vi "20180801 2nd Step Analysis.vi"(8 "error in":errorcluster caption="エラー入力（エラーなし）", 9 "Numeric":i32=5, 10 "S New Info and MiN":T28={"Sample Sequence"="GATGATGATGATGATGAT", "Right Read MIN"=6, "Filter P"=0, "STD Type"=enum."Region", "Base Table"=[], "Selection"=enum."10kHz", "noise MAX"=3, "Sample name"="(GAT)x6"} {"Base Table"."Value 3" format="%.2g"}, 11 "Filename":path) -> (0 "error out":errorcluster caption="エラー出力", 2 "Raw data Graph":dbl[](graph), 3 "Total NGraph_MS":dbl[][](graph))   [LabVIEW 2018]
uses:
  VI/control1.ctl
  <vilib>/Analysis/NI_AALBase.lvlib
panel:
  out "error out 3":errorcluster
  out "FN#":string
  out "Array":string[](array[string])
  out "error out 2":errorcluster caption="エラー出力"
  in  "target path (use dialog)":path
  out "B_TDMS_Path_Temp":path
  out "MS_Total Con and T":cluster{dbl[], dbl[], dbl[], dbl[], i32[]}
  out "Plot Graph":dbl[][](graph)
  out "Base_Tag_Array":string[](array[string])
  out "Base_Com_Array":i32[](array[numeric])
  out "Total C Plot_MS":dbl[][](array[numeric])
  out "R Con H_MS":dbl[][](array[numeric])
  out "LCPZ":T1
  out "LCPX_CZ":T1
  out "LCPX_C2":T2
  out "LAP Table":string[][](table) caption="LCP Table"
  out "Table cluster_B":T3
  out "LSP_C2":T4
  out "LSPX_C1":T5
  out "LCPX_C1":T6
  out "Assigned#_CL":T4
  out "AR BN#":i32[](array[numeric])
  out "Long Signal#":i32
  out "AR T#":i32
  in  "B_END [s]":dbl format="%#_13g"
  in  "B_Start [s]":dbl format="%#_13g"
  in  "Tag cluster_B":T7
  out "LTP Table":string[][](table) caption="LS Table"
  out "LTP Table Tag":string[](array[string])
  out "LTP Table Pass":path
  out "MxRight_Array":string[](array[string])
  out "Assigned_Array":string[](array[string])
  out "LSP_C2":T8
  out "LSP_C1":T9
  in  "LCP_C1":T10
  out "LCP Table CSV refnum":refnum<file>
  out "LSP Table CSV refnum":refnum<file>
  out "LSP Table":string[][](table) caption="LS Table"
  out "LCP Table":string[][](table) caption="CP Table"
  out "LCP Table Tag":string[](array[string])
  out "LSP Table Tag":string[](array[string])
  out "LCP Table Pass":path
  out "LSP Table Pass":path
  out "after":string
  out "BNAL TD":T11
  out "BNAL Program Date":string
  out "B prep":T12
  out "BNAL Program":string
  out "TDMS Tpath":refnum<k34>
  out "AR Table":string[][](array[string])
  out "AR Table Tag":string[](array[string])
  out "S Table Tag":string[](array[string])
  out "B_TDMS_Path":path
  out "B_TDMS Path":string
  out "BR time [s]":dbl
  out "assembly C":T13 {"Assembly Ratio" format="%#.2g"}
  out "GAF":T14
  in  "noise MAX":i32=3
  out "AR#":i32[](array[numeric])
  out "RR#":i32[](array[numeric])
  out "Anal Time":string
  out "1s datapoint":i32
  in  "Selection":enum16{"10kHz", "100kHz"}(ring)
  out "BR all info":T15
  out "B info":string[](array[string])
  out "AC Table Tag":string[](array[string])
  out "R Table Tag":string[](array[string])
  out "R Con H":dbl[][](array[numeric])
  out "BC1":cluster{"B region#":i32, "Date":string}
  out "BNAL Path":T16
  out "LS Path":T17
  out "Total C Plot":dbl[][](graph)
  out "Folder Path":string
  out "Date":string
  out "Base R Level":dbl[](array[numeric])
  out "Base A Level":dbl[](array[numeric])
  out "Base Color":u32[](array[numeric])
  out "Level Composition":string[](array[string])
  out "Base Ex Info":T18
  out "Total Con and T":T19
  out "CP A Tag AZ":string[](array[string])
  out "Time A Table AZ":string[](array[string])
  out "BS Table Tag":string[](array[string])
  out "BS Table":string[][](table) caption="S Table"
  out "GR data":T20
  out "Selected Raw D":T21
  in  "Control_2":T22(tab)
  out "Time Graph":cluster{"time":dbl[], "current":dbl[]}[](graph)
  out "Time Graph Profile":cluster{"time":dbl[], dbl[]}[](graph)
  out "Label":T23
  out "CP Graph":cluster{i32[], dbl[]}[](graph)
  out "CP Graph Profile":cluster{i32[], dbl[]}[](graph)
  out "Label 2":T23
  out "Signal# Histogram":cluster{"配列 2":i32[], "配列 5":dbl[]}[](graph)
  out "Long Assembly":bool[][](array[boolean])
  out "Total assembly C":T24 {"Assembly Ratio 2" format="%#_3g"; "Assembly Ratio" format="%#_3g"}
  out "Total BC":bool[](array[boolean])
  out "RR#":i32
  out "S#":i32
  out "Av R_Read N":dbl format="%#_4g"
  out "Av N_Read N":dbl format="%#_4g"
  out "Covered?":bool
  out "MAX RR#":i32
  out "coverage [%]":dbl format="%#.2g"
  out "5’→3'":dbl format="%#.3g"
  out "Total Base CP":i32
  out "RR MIN Over S#":i32
  out "SB_ANA":T25
  out "Av n#bp":i32
  out "Av RR n#bp":i32
  out "Av RRn# kbp/day":dbl format="%#_3f"
  out "Av n# kbp/day":dbl format="%#_3f"
  out "Total AGraph":dbl[][](graph)
  out "Q_Histogram":T26(graph)
  out "Time Histogram":T26(graph)
  out "I Histogram":T26(graph) caption="I_Histogram"
  out "Total NGraph":dbl[][](graph)
  out "Count Graph":cluster{i32[], i32[]}(graph) caption="ヒストグラムグラフ"
  out "Cutted Sample Sequence":string
  out "MS_Count Graph":cluster{i32[], i32[]}(graph) caption="ヒストグラムグラフ"
  out "Sample Sequence":string
  out "All Radar_X":picture
  out "All Radar Plot_XX":picture
  out "Mono Table":string[][](table)
  out "Di Table":string[][](table)
  out "Tri Table":string[][](table)
  out "Base Species (n)":i32
  out "Right Read MIN":i32
  out "Base (n)":i32
  in  "Control_1":T27(tab)
  in  "Locked":bool=TRUE
  out "before":string
  out "B Table":string[][](table)
  out "R Table":string[][](table)
  out "Data Histogram":T26(graph) caption="ヒストグラムグラフ"
  out "Label 3":T23
  out "AC Table":T29
  out "Progress":dbl(slide) scale=0.0..100.0
  out "B_Region#":i32
  out "Total B Region#":i32
  out "Channel Tag":string[](array[string])
  out "Table Tag":string[][](array[string])
  out "B End [s]":dbl[](array[numeric])
  out "B Start [s]":dbl[](array[numeric])
  out "B Table Tag":string[](array[string])
  out "Raw data":dbl[](array[numeric])
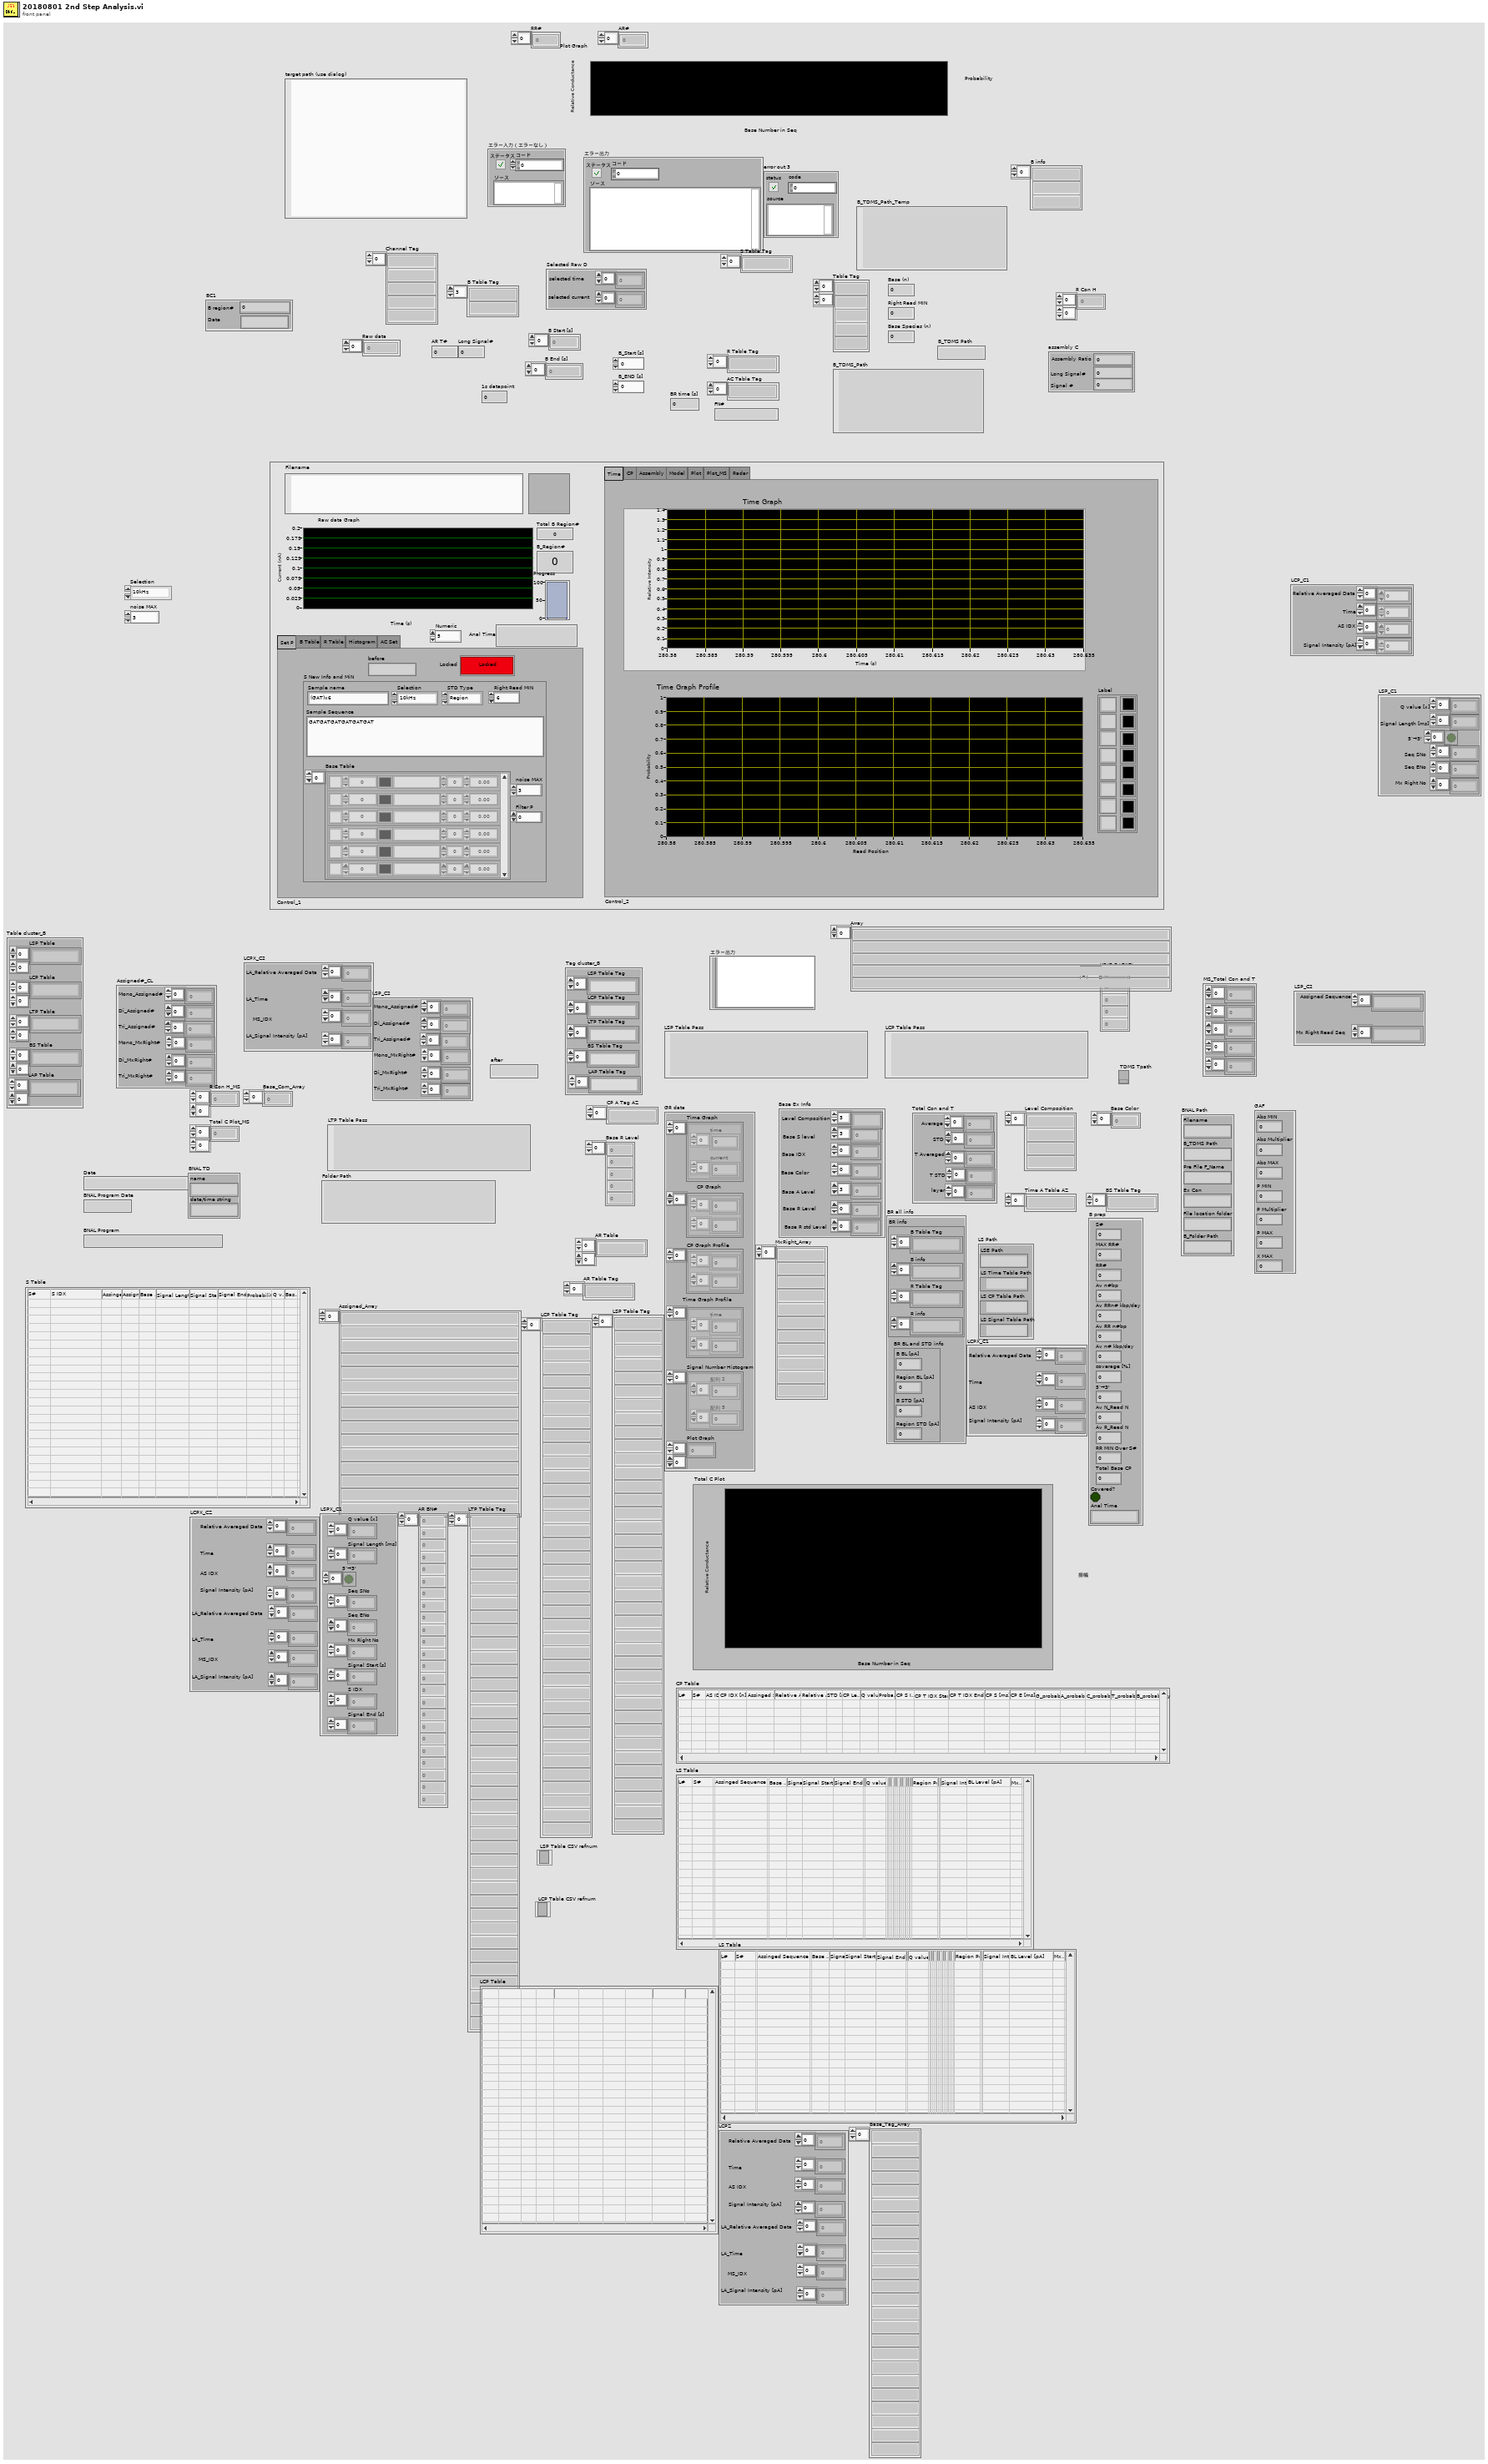
[diagram p1: front panel]
types:
  T1 = cluster{"Relative Averaged Data":dbl[], "Time":dbl[], "AS IDX":i32[], "Signal Intensity [pA]":dbl[], "LA_Relative Averaged Data":dbl[], "LA_Time":dbl[], "MS_IDX":i32[], "LA_Signal Intensity [pA]":dbl[]}
  T2 = cluster{"LA_Relative Averaged Data":dbl[], "LA_Time":dbl[], "MS_IDX":i32[], "LA_Signal Intensity [pA]":dbl[]}
  T3 = cluster{"LSP Table":string[][], "LCP Table":string[][], "LTP Table":string[][], "BS Table":string[][], "LAP Table":string[][]}
  T4 = cluster{"Mono_Assigned#":i32[], "Di_Assigned#":i32[], "Tri_Assigned#":i32[], "Tri_MxRight#":i32[], "Di_MxRight#":i32[], "Mono_MxRight#":i32[]}
  T5 = cluster{"Q value [x]":dbl[], "Signal Length [ms]":dbl[], "5’→3'":bool[], "Seq SNo":i32[], "Seq ENo":i32[], "Mx Right No":i32[], "Signal Start [s]":dbl[], "S IDX":i32[], "Signal End [s]":dbl[]}
  T6 = cluster{"Relative Averaged Data":dbl[], "Time":dbl[], "AS IDX":i32[], "Signal Intensity [pA]":dbl[]}
  T7 = cluster{"LSP Table Tag":string[], "LCP Table Tag":string[], "LTP Table Tag":string[], "BS Table Tag":string[], "LAP Table Tag":string[]}
  T8 = cluster{"Assigned Sequence":string[], "Mx Right Read Seq":string[]}
  T9 = cluster{"Q value [x]":dbl[], "Signal Length [ms]":dbl[], "5’→3'":bool[], "Seq SNo":i32[], "Seq ENo":i32[], "Mx Right No":i32[]}
  T10 = cluster{"Relative Averaged Data":dbl[], "Time":dbl[], i32[], "Signal Intensity [pA]":dbl[]}
  T11 = cluster{"name":string, "date/time string":string}
  T12 = cluster{"S#":i32, "MAX RR#":i32, "RR#":i32, "Av n#bp":i32, "Av RRn# kbp/day":dbl, "Av RR n#bp":i32, "Av n# kbp/day":dbl, "coverage [%]":dbl, "5’→3'":dbl, "Av N_Read N":dbl, "Av R_Read N":dbl, "RR MIN Over S#":i32, "Total Base CP":i32, "Covered?":bool, "Anal Time":string}
  T13 = cluster{"Assembly Ratio":dbl, "Long Signal#":i32, "Signal #":i32}
  T14 = cluster{"Abs MIN":dbl, "Abs Multiplier":dbl, "Abs MAX":dbl, "P MIN":dbl, "P Multiplier":dbl, "P MAX":dbl, "X MAX":dbl}
  T15 = cluster{"BR info":cluster{"B Table Tag":string[], "B info":string[], "R Table Tag":string[], "R info":string[]}, "BR BL and STD info":cluster{"B BL [pA]":dbl, "Region BL [pA]":dbl, "B STD [pA]":dbl, "Region STD [pA]":dbl}}
  T16 = cluster{"Filename":string, "B_TDMS Path":string, "Pre File F_Name":string, "Ex Con":string, "File location folder":string, "B_Folder Path":string}
  T17 = cluster{"LSE Path":string, "LS Time Table Path":path, "LS CP Table Path":path, "LS Signal Table Path":path}
  T18 = cluster{"Level Composition":string[], "Base S level":dbl[], "Base IDX":i32[], "Base Color":u32[], "Base A Level":dbl[], "Base R Level":dbl[], "Base R std Level":dbl[]}
  T19 = cluster{"Average":dbl[], "STD":dbl[], "T Averaged":dbl[], "T STD":dbl[], "layer":i32[]}
  T20 = cluster{"Time Graph":cluster{"time":dbl[], "current":dbl[]}[], "CP Graph ":cluster{i32[], dbl[]}[], "CP Graph Profile":cluster{i32[], dbl[]}[], "Time Graph Profile":cluster{"time":dbl[], dbl[]}[], "Signal Number Histogram":cluster{"配列 2":i32[], "配列 5":dbl[]}[], "Plot Graph":dbl[][]}
  T21 = cluster{"selected time":dbl[], "selected current":dbl[]}
  T22 = enum32{"Time", "CP", "Assembly", "Model", "Plot", "Plot_MS", "Radar"}
  T23 = cluster{"カラーボックス":u32, "カラーボックス 4":u32, "カラーボックス 2":u32, "カラーボックス 5":u32, "カラーボックス 3":u32, "カラーボックス 6":u32, "カラーボックス 7":u32, "カラーボックス 8":u32, "B0":string, "B1":string, "B2":string, "B3":string, "B4":string, "B5":string, "B6":string, "B7":string}
  T24 = cluster{"Assembly Ratio":dbl, "Long Signal#":i32, "Signal #":i32, "Assembly Ratio 2":dbl}
  T25 = cluster{"RR Ratio (%)":dbl, "Base Species#":i32, "RR option#":i32, "all option#":i32, "RRS#":i32, "Base Cutted Q#":i32}
  T26 = cluster{"X Values":dbl[], "Histogram: h(x)":i32[]}
  T27 = enum32{"Set P", "B Table", "R Table", "Histogram", "AC Set"}
  T28 = cluster{"Sample Sequence":string, "Right Read MIN":i32, "Filter P":i32, "STD Type":enum16{"Region", "Each", "Fixed"}, "Base Table":cluster{"Name":string, "Value":dbl, "Color":u32, "Name 2":string, "Value 2":dbl, "Value 3":dbl}[], "Selection":enum16{"10kHz", "100kHz"}, "noise MAX":i32, "Sample name":string}
  T29 = typedef "control1.ctl" = string[][]
  T30 = cluster{"Relative Averaged Data":dbl[], "Time":dbl[], "AS IDX":i32[], "Abs Average":dbl[]}
  T31 = enum16{"open", "open or create", "create or replace", "create", "open (read-only)"}
  T32 = cluster{"Name":string, "Value":dbl, "Color":u32, "Name 2":string, "Value 2":dbl, "Value 3":dbl}[]
  T33 = cluster{"Base Composition":string[], "Base S Level":dbl[], "Color IDX":u32[], "Base ex Composition":string[], "Base IDX":i32[], "STD S Level [pA]":dbl[]}
  T34 = cluster{"Assembly Ratio":dbl, "Assembly Ratio":i32, "Assembly Ratio":i32, "Assembly Ratio":dbl}
  T35 = cluster{"LSP Table Pass":path, "LCP Table Pass":path, "LTP Table Pass":path}
  T36 = cluster{"Data Estimated Info":cluster{"Mx level":dbl, "Mx Level Intensity":dbl, "BL Level":dbl, "MAX":dbl, "Min":dbl, "Histogram bin":dbl, "Region Cut":dbl, "Data Point":i32, "Filename":string, "G level intensity":dbl}, "Base Ex Info":cluster{"Level Composition":string[], "Base S level":dbl[], "Base IDX":i32[], "Base Color":u32[], "Base A Level":dbl[], "Base R Level":dbl[], "Base R std Level":dbl[]}}
  T37 = cluster{"Assigned Sequence":string[], "L#":i32[], "Mx Right Read Seq":string[], "Base Number":i32[], "Signal Intensity [pA]":dbl[]}
  T38 = cluster{"Count Graph":cluster{i32[], i32[]}, "Total Con and T":cluster{dbl[], dbl[], dbl[], dbl[], i32[]}, "GAT":cluster{"Value":cluster{"Abs MIN":dbl, "Abs Multiplier":dbl, "Abs MAX":dbl, "P MIN":dbl, "P Multiplier":dbl, "P MAX":dbl, "X MAX":dbl}, "Axis":dbl[], "Axis":dbl[]}}
  T39 = cluster{"Plot Graph":dbl[][], "N_Grpah":dbl[][], "Abs_Graph":dbl[][]}
  T40 = cluster{"Value":cluster{"Abs MIN":dbl, "Abs Multiplier":dbl, "Abs MAX":dbl, "P MIN":dbl, "P Multiplier":dbl, "P MAX":dbl, "X MAX":dbl}, "Axis":dbl[], "Axis":dbl[]}
  T41 = cluster{"Mono Table":string[][], "Mono Table":string[][], "Mono Table":string[][]}
  T42 = cluster{"Radar Plot":picture, "Radar Plot":picture, "Radar Plot":picture}
  T43 = cluster{"Value":i32, "Value":i32, "Value":i32, "Value":i32, "Value":dbl, "Value":i32, "Value":dbl, "Value":dbl, "Value":dbl, "Value":dbl, "Value":dbl, "Value":i32, "Value":i32, "Value":bool, "Value":string}
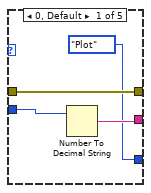
[diagram p3: hidden frame]
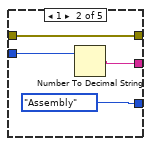
[diagram p4: hidden frame]
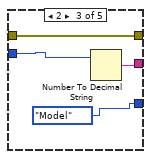
[diagram p5: hidden frame]
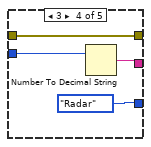
[diagram p6: hidden frame]
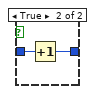
[diagram p7: hidden frame]
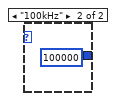
[diagram p9: hidden frame]
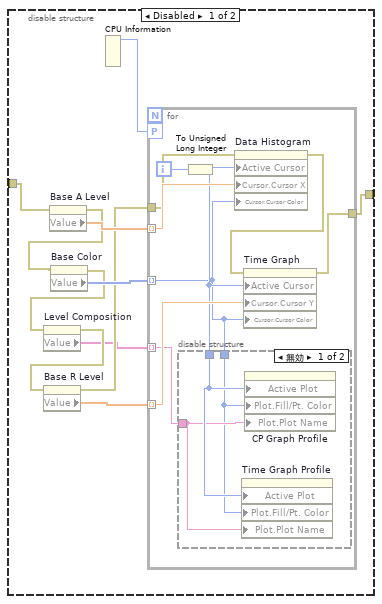
[diagram p10: hidden frame]
diagram:
  w25 = FALSE ("entire hierarchy (F)")
  w95 = T1 {"Relative Averaged Data"=[], "Time"=[], "AS IDX"=[], "Signal Intensity [pA]"=[], "LA_Relative Averaged Data"=[], "LA_Time"=[], "MS_IDX"=[], "LA_Signal Intensity [pA]"=[]} ("LCPZ")
  w162 = 86.4 ("y")
  w212 = T4 {"Mono_Assigned#"=[0, 0, 0, 0, 0, 0, 0, 0, 0, 0, 0, 0, 0, 0, 0, 0, 0, 0, 0, 0, 0, 0, 0, 0, 4, 3, 2, 2, 4, 2, 2, 2, 1, 3, 3, 6, 0, 0, 0, 0, 0, 35, 41, 19, 12, 25, 36, 30, 11, 12, 7, 8, 4, 4, 6, 5, 0, 0, 0, 0, 1, 30, 41, 18, 0, 3, 9, 10, 5, 24, 45, 26, 0, 0, 0, 0, 4, 4, 4, 4, 4, 4, 4, 4, 2, 4, 17, 15, 0, 0, 0, 0, 1, 2, 2, 4, 0, 0, 0, 0, 2, 2, 1, 3, 9, 16, 15, 14, 0, 0, 0, 0, 4, 14, 13, 17, 1, 19, 47, 49, 0, 4, 8, 7, 0, 2, 5, 4, 0, 0, 0, 0, 0, 8, 12, 10, 1, 8, 9, 13, 0, 4, 4, 5, 0, 0, 0, 0, 1, 1, 3, 3, 1, 14, 14, 18, 1, 10, 13, 17, 4, 9, 17, 17, 13, 30, 35, 36, 4, 20, 24, 15, 0, 0, 0, 0, 9, 15, 9, 15, 1, 1, 5, 5, 3, 4, 2, 3, 0, 0, 0, 0, 0, 0, 0, 0, 8, 24, 28, 35, 2, 5, 6, 7, 8, 13, 11, 18, 0, 10, 9, 14, 2, 8, 4, 6, 3, 79, 114, 73, 0, 2, 7, 6, 0, 3, 5, 4, 0, 0, 0, 0, 7, 20, 27, 23, 0, 0, 0, 0, 4, 8, 7, 5, 9, 35, 30, 24, 24, 58, 51, 32, 0, 0, 0, 0, 4, 9, 15, 15, 0, 0, 0, 0, 5, 45, 47, 43, 3, 13, 21, 19, 0, 0, 0, 0, 21, 51, 44, 39, 0, 0, 0, 0, 3, 7, 11, 15, 0, 0, 0, 0, 10, 25, 39, 42, 0, 0, 0, 0, 8, 16, 21, 23, 1, 1, 2, 3, 0, 0, 0, 0, 5, 7, 11, 12, 6, 24, 17, 21, 41, 59, 28, 32, 47, 75, 40, 46, 0, 0, 0, 0, 81, 119, 96, 69, 8, 10, 6, 2, 1, 2, 2, 3, 9, 19, 10, 12, 8, 12, 11, 14, 13, 50, 67, 73, 19, 16, 5, 8, 11, 21, 19, 13, 5, 7, 2, 2, 0, 9, 22, 29, 0, 0, 0, 0, 2, 26, 79, 77, 20, 27, 15, 8, 0, 0, 0, 0, 0, 0, 0, 0, 6, 6, 2, 3, 17, 18, 5, 3, 18, 42, 29, 6, 6, 8, 6, 7, 3, 4, 5, 3, 0, 0, 0, 0, 1, 4, 5, 7, 9, 33, 35, 19, 11, 16, 16, 9, 5, 42, 42, 48, 15, 57, 57, 53, 13, 18, 8, 14, 16, 28, 21, 16, 6, 5, 6, 4, 12, 18, 11, 6, 0, 0, 0, 0, 0, 0, 0, 0, 2, 2, 2, 3, 0, 0, 0, 0, 0, 0, 0, 0, 8, 58, 83, 59, 7, 18, 17, 19, 19, 42, 46, 47, 26, 56, 61, 34, 12, 20, 26, 17, 4, 4, 4, 6, 15, 24, 24, 15, 26, 43, 32, 27, 11, 11, 5, 2, 4, 27, 28, 24, 5, 6, 2, 4, 4, 6, 9, 7, 6, 15, 15, 21, 13, 31, 40, 44, 0, 0, 0, 0, 0, 0, 0, 0, 1, 2, 3, 5, 0, 0, 0, 0, 17, 25, 18, 6, 0, 0, 0, 0, 0, 0, 0, 0, 0, 0, 0, 0, 0, 0, 0, 0, 0, 0, 0, 0, 0, 0, 0, 0, 0, 0, 0, 0, 0, 0, 0, 0, 4, 3, 2, 2, 4, 2, 2, 2, 1, 3, 3, 6, 0, 0, 0, 0, 0, 35, 41, 19, 12, 25, 36, 30, 11, 12, 7, 8, 4, 4, 6, 5, 0, 0, 0, 0, 1, 30, 41, 18, 0, 3, 9, 10, 5, 24, 45, 26, 0, 0, 0, 0, 4, 4, 4, 4, 4, 4, 4, 4, 2, 4, 17, 15, 0, 0, 0, 0, 1, 2, 2, 4], "Di_Assigned#"=[0, 0, 0, 0, 0, 0, 0, 0, 0, 0, 0, 0, 0, 0, 0, 0, 0, 0, 0, 0, 0, 0, 0, 0, 0, 0, 0, 0, 0, 0, 0, 0, 0, 0, 0, 0, 0, 0, 0, 0, 0, 0, 0, 0, 0, 0, 0, 0, 0, 0, 0, 0, 0, 0, 0, 0, 0, 0, 0, 0, 0, 0, 0, 0, 0, 0, 0, 0, 0, 0, 0, 0, 1, 2, 0, 1, 1, 0, 1, 1, 1, 1, 0, 1, 0, 2, 0, 1, 1, 0, 0, 2, 1, 1, 0, 1, 0, 0, 3, 1, 0, 1, 0, 0, 1, 2, 3, 1, 0, 0, 0, 0, 0, 0, 0, 0, 0, 0, 0, 0, 28, 0, 7, 30, 0, 11, 0, 0, 0, 5, 13, 0, 9, 10, 6, 15, 1, 18, 6, 3, 3, 4, 23, 1, 3, 5, 4, 1, 4, 2, 9, 1, 1, 2, 2, 2, 2, 1, 1, 2, 2, 1, 0, 3, 1, 2, 1, 1, 0, 0, 0, 0, 0, 0, 0, 0, 0, 0, 0, 0, 26, 0, 3, 26, 0, 15, 1, 0, 0, 3, 14, 1, 1, 0, 2, 2, 0, 7, 0, 0, 0, 1, 8, 0, 17, 4, 3, 21, 1, 22, 2, 3, 0, 1, 25, 0, 0, 0, 0, 0, 0, 0, 0, 0, 0, 0, 0, 0, 1, 2, 1, 1, 1, 2, 2, 1, 1, 1, 1, 1, 1, 2, 1, 1, 1, 2, 2, 1, 1, 1, 1, 1, 2, 2, 0, 2, 0, 15, 1, 1, 0, 1, 13, 0, 0, 0, 0, 0, 0, 0, 0, 0, 0, 0, 0, 0, 1, 0, 1, 0, 0, 2, 1, 0, 0, 1, 1, 1, 0, 0, 0, 0, 0, 0, 0, 0, 0, 0, 0, 0, 0, 2, 0, 1, 0, 0, 0, 0, 2, 1, 1, 0, 6, 6, 4, 5, 2, 7, 7, 1, 0, 4, 8, 1, 0, 0, 0, 0, 0, 0, 0, 0, 0, 0, 0, 0, 4, 2, 8, 3, 1, 8, 3, 1, 0, 8, 5, 1, 9, 1, 9, 9, 0, 38, 1, 0, 0, 9, 37, 0, 3, 0, 1, 3, 0, 5, 0, 0, 0, 1, 4, 0, 2, 0, 0, 1, 0, 4, 0, 0, 0, 1, 2, 0, 0, 0, 0, 0, 0, 0, 0, 0, 0, 0, 0, 0, 5, 0, 3, 6, 0, 5, 0, 0, 0, 2, 7, 0, 2, 0, 6, 3, 1, 5, 0, 1, 0, 5, 6, 0, 2, 0, 2, 3, 0, 1, 0, 0, 0, 1, 2, 0, 0, 0, 0, 0, 0, 0, 0, 0, 0, 0, 0, 0, 1, 0, 0, 1, 1, 1, 0, 0, 1, 0, 2, 0, 7, 1, 6, 5, 0, 9, 1, 0, 0, 8, 6, 0, 5, 0, 5, 2, 1, 10, 1, 0, 0, 7, 7, 0, 7, 2, 0, 2, 1, 14, 1, 2, 1, 6, 8, 1, 11, 10, 9, 10, 2, 23, 11, 0, 2, 9, 24, 1, 14, 3, 3, 14, 0, 10, 4, 0, 0, 2, 10, 1, 0, 0, 0, 0, 0, 0, 0, 0, 0, 0, 0, 0, 2, 7, 6, 3, 1, 5, 7, 0, 2, 5, 7, 1, 0, 0, 1, 0, 1, 3, 1, 0, 0, 0, 5, 0, 1, 2, 1, 0, 1, 1, 2, 1, 0, 2, 0, 0, 0, 0, 0, 0, 0, 0, 0, 0, 0, 0, 0, 0, 0, 0, 0, 0, 0, 0, 0, 0, 0, 0, 0, 0, 5, 3, 14, 8, 2, 17, 3, 2, 2, 12, 19, 3, 0, 1, 4, 2, 1, 3, 1, 0, 0, 2, 5, 0, 2, 1, 10, 2, 2, 5, 2, 5, 1, 9, 4, 4, 3, 0, 7, 3, 0, 6, 0, 0, 0, 6, 6, 0, 2, 1, 4, 4, 0, 0, 1, 0, 1, 3, 2, 1, 62, 1, 15, 60, 0, 54, 3, 0, 0, 15, 50, 2, 2, 0, 0, 2, 0, 5, 0, 0, 0, 0, 5, 0, 2, 0, 1, 3, 0, 2, 0, 0, 0, 0, 3, 0, 0, 0, 0, 0, 0, 0, 0, 0, 0, 0, 0, 0, 9, 5, 6, 12, 1, 14, 4, 2, 1, 4, 16, 1, 0, 0, 0, 0, 0, 0, 0, 0, 0, 0, 0, 0, 5, 2, 1, 3, 0, 3, 3, 0, 1, 2, 2, 1, 18, 5, 12, 18, 1, 10, 6, 2, 1, 10, 9, 3, 31, 11, 16, 30, 11, 9, 15, 4, 5, 12, 14, 2, 0, 0, 0, 0, 0, 0, 0, 0, 0, 0, 0, 0, 4, 1, 4, 4, 2, 8, 0, 2, 2, 5, 7, 1, 0, 0, 0, 0, 0, 0, 0, 0, 0, 0, 0, 0, 23, 3, 18, 22, 1, 23, 1, 3, 1, 22, 19, 1, 7, 2, 4, 7, 1, 12, 1, 1, 1, 5, 12, 0, 0, 0, 0, 0, 0, 0, 0, 0, 0, 0, 0, 0, 20, 14, 17, 20, 5, 19, 12, 7, 2, 18, 17, 2, 0, 0, 0, 0, 0, 0, 0, 0, 0, 0, 0, 0, 3, 1, 3, 1, 1, 9, 0, 0, 3, 5, 8, 0, 0, 0, 0, 0, 0, 0, 0, 0, 0, 0, 0, 0, 9, 4, 11, 10, 2, 26, 3, 4, 3, 11, 26, 4, 0, 0, 0, 0, 0, 0, 0, 0, 0, 0, 0, 0, 3, 6, 7, 4, 2, 14, 5, 3, 0, 7, 15, 0, 0, 0, 1, 0, 1, 1, 0, 1, 0, 1, 1, 0, 0, 0, 0, 0, 0, 0, 0, 0, 0, 0, 0, 0, 2, 4, 1, 0, 1, 10, 4, 1, 0, 3, 8, 0, 10, 5, 9, 10, 0, 6, 2, 0, 3, 11, 7, 1, 12, 37, 10, 9, 2, 17, 35, 3, 3, 15, 12, 2, 17, 42, 16, 16, 2, 22, 37, 4, 6, 21, 18, 3, 0, 0, 0, 0, 0, 0, 0, 0, 0, 0, 0, 0, 36, 70, 11, 36, 9, 51, 66, 10, 5, 16, 49, 2, 2, 7, 0, 4, 1, 1, 4, 3, 1, 2, 0, 0, 1, 1, 0, 1, 0, 1, 0, 0, 1, 1, 1, 0, 4, 9, 6, 6, 0, 2, 7, 1, 1, 5, 5, 0, 2, 5, 5, 6, 1, 4, 3, 1, 4, 3, 8, 2, 18, 10, 21, 16, 1, 47, 7, 2, 4, 26, 42, 2, 2, 11, 1, 0, 3, 2, 12, 3, 4, 3, 0, 3, 10, 7, 4, 10, 3, 5, 7, 2, 2, 3, 7, 1, 2, 4, 0, 2, 0, 0, 4, 0, 1, 1, 0, 1, 1, 0, 8, 2, 0, 20, 0, 0, 0, 7, 21, 0, 0, 0, 0, 0, 0, 0, 0, 0, 0, 0, 0, 0, 16, 0, 10, 11, 1, 67, 0, 2, 0, 15, 60, 1, 9, 16, 1, 6, 2, 5, 14, 4, 2, 4, 2, 2, 0, 0, 0, 0, 0, 0, 0, 0, 0, 0, 0, 0, 0, 0, 0, 0, 0, 0, 0, 0, 0, 0, 0, 0, 1, 5, 0, 0, 1, 1, 5, 0, 1, 1, 1, 0, 4, 13, 1, 2, 3, 0, 14, 1, 2, 2, 0, 0, 24, 16, 2, 23, 2, 4, 15, 3, 0, 3, 2, 0, 2, 4, 2, 2, 1, 3, 4, 1, 1, 2, 3, 1, 3, 1, 0, 1, 2, 2, 2, 1, 0, 1, 1, 0, 0, 0, 0, 0, 0, 0, 0, 0, 0, 0, 0, 0, 1, 0, 3, 1, 1, 3, 1, 0, 0, 2, 4, 0, 22, 3, 8, 22, 3, 9, 5, 3, 1, 6, 10, 3, 10, 3, 2, 8, 3, 5, 4, 5, 2, 4, 1, 4, 18, 3, 21, 17, 0, 22, 4, 1, 0, 21, 21, 2, 28, 3, 25, 30, 6, 20, 3, 5, 7, 23, 24, 6, 6, 7, 4, 3, 1, 4, 8, 0, 5, 7, 1, 5, 12, 7, 8, 11, 5, 4, 10, 6, 0, 6, 2, 4, 3, 2, 0, 1, 3, 1, 3, 1, 2, 1, 2, 1, 8, 7, 2, 6, 3, 2, 8, 2, 2, 3, 1, 1, 0, 0, 0, 0, 0, 0, 0, 0, 0, 0, 0, 0, 0, 0, 0, 0, 0, 0, 0, 0, 0, 0, 0, 0, 0, 1, 1, 1, 0, 1, 0, 1, 1, 1, 1, 0, 0, 0, 0, 0, 0, 0, 0, 0, 0, 0, 0, 0, 0, 0, 0, 0, 0, 0, 0, 0, 0, 0, 0, 0, 37, 2, 19, 38, 6, 38, 3, 4, 1, 17, 42, 0, 5, 5, 8, 7, 1, 9, 4, 2, 1, 7, 10, 1, 12, 9, 20, 20, 5, 19, 5, 8, 6, 16, 25, 5, 32, 8, 15, 32, 11, 17, 8, 15, 2, 13, 12, 7, 11, 7, 2, 9, 5, 12, 9, 2, 1, 2, 13, 0, 0, 2, 2, 0, 0, 4, 3, 1, 0, 1, 2, 2, 13, 5, 5, 12, 7, 4, 4, 5, 6, 7, 4, 3, 21, 11, 10, 20, 7, 4, 10, 7, 9, 13, 4, 8, 3, 7, 1, 3, 2, 0, 8, 1, 1, 0, 0, 2, 16, 2, 9, 16, 1, 11, 0, 1, 3, 10, 11, 1, 2, 4, 0, 1, 0, 1, 4, 0, 1, 1, 0, 1, 4, 1, 1, 1, 2, 5, 2, 2, 0, 3, 3, 1, 7, 2, 5, 3, 1, 11, 2, 2, 2, 10, 6, 3, 11, 6, 13, 14, 2, 23, 2, 4, 7, 14, 24, 5, 0, 0, 0, 0, 0, 0, 0, 0, 0, 0, 0, 0, 0, 0, 0, 0, 0, 0, 0, 0, 0, 0, 0, 0, 1, 0, 1, 1, 0, 2, 0, 0, 1, 1, 2, 1, 0, 0, 0, 0, 0, 0, 0, 0, 0, 0, 0, 0, 11, 10, 4, 13, 5, 0, 10, 6, 1, 2, 1, 2, 0, 0, 0, 0, 0, 0, 0, 0, 0, 0, 0, 0, 0, 0, 0, 0, 0, 0, 0, 0, 0, 0, 0, 0, 0, 0, 0, 0, 0, 0, 0, 0, 0, 0, 0, 0, 0, 0, 0, 0, 0, 0, 0, 0, 0, 0, 0, 0, 0, 0, 0, 0, 0, 0, 0, 0, 0, 0, 0, 0, 0, 0, 0, 0, 0, 0, 0, 0, 0, 0, 0, 0, 0, 0, 0, 0, 0, 0, 0, 0, 0, 0, 0, 0, 0, 0, 0, 0, 0, 0, 0, 0, 0, 0, 0, 0, 1, 2, 0, 1, 1, 0, 1, 1, 1, 1, 0, 1, 0, 2, 0, 1, 1, 0, 0, 2, 1, 1, 0, 1, 0, 0, 3, 1, 0, 1, 0, 0, 1, 2, 3, 1, 0, 0, 0, 0, 0, 0, 0, 0, 0, 0, 0, 0, 28, 0, 7, 30, 0, 11, 0, 0, 0, 5, 13, 0, 9, 10, 6, 15, 1, 18, 6, 3, 3, 4, 23, 1, 3, 5, 4, 1, 4, 2, 9, 1, 1, 2, 2, 2, 2, 1, 1, 2, 2, 1, 0, 3, 1, 2, 1, 1, 0, 0, 0, 0, 0, 0, 0, 0, 0, 0, 0, 0, 26, 0, 3, 26, 0, 15, 1, 0, 0, 3, 14, 1, 1, 0, 2, 2, 0, 7, 0, 0, 0, 1, 8, 0, 17, 4, 3, 21, 1, 22, 2, 3, 0, 1, 25, 0, 0, 0, 0, 0, 0, 0, 0, 0, 0, 0, 0, 0, 1, 2, 1, 1, 1, 2, 2, 1, 1, 1, 1, 1, 1, 2, 1, 1, 1, 2, 2, 1, 1, 1, 1, 1, 2, 2, 0, 2, 0, 15, 1, 1, 0, 1, 13, 0, 0, 0, 0, 0, 0, 0, 0, 0, 0, 0, 0, 0, 1, 0, 1, 0, 0, 2, 1, 0, 0, 1, 1, 1], "Tri_Assigned#"=array[5868 elements], "Tri_MxRight#"=[0, 0, 0, 0, 0, 0, 0, 0, 0, 0, 0, 0, 0, 0, 0, 0, 0, 0, 0, 0, 0, 0, 0, 0, 2, 2, 1, 1, 2, 2, 1, 1, 1, 2, 1, 3, 0, 0, 0, 0, 0, 2, 3, 2, 2, 10, 9, 7, 3, 5, 3, 3, 1, 3, 4, 4, 0, 0, 0, 0, 0, 2, 3, 1, 0, 2, 3, 2, 0, 2, 3, 2, 0, 0, 0, 0, 3, 2, 2, 0, 3, 2, 2, 0, 0, 2, 2, 2, 0, 0, 0, 0, 1, 2, 1, 3, 0, 0, 0, 0, 2, 2, 0, 2, 1, 6, 5, 7, 0, 0, 0, 0, 1, 7, 7, 10, 1, 7, 5, 6, 0, 4, 4, 4, 0, 2, 2, 2, 0, 0, 0, 0, 0, 4, 5, 4, 0, 4, 3, 6, 0, 4, 4, 5, 0, 0, 0, 0, 1, 1, 3, 1, 0, 8, 7, 9, 1, 6, 3, 8, 3, 3, 3, 4, 2, 6, 3, 4, 0, 4, 5, 3, 0, 0, 0, 0, 5, 5, 0, 2, 1, 1, 2, 2, 2, 4, 1, 1, 0, 0, 0, 0, 0, 0, 0, 0, 3, 11, 8, 12, 1, 2, 1, 2, 3, 7, 2, 6, 0, 5, 2, 5, 1, 3, 1, 1, 0, 15, 17, 12, 0, 2, 3, 1, 0, 2, 3, 1, 0, 0, 0, 0, 2, 4, 4, 3, 0, 0, 0, 0, 0, 2, 2, 2, 3, 7, 5, 5, 4, 13, 8, 9, 0, 0, 0, 0, 4, 4, 5, 6, 0, 0, 0, 0, 2, 7, 6, 5, 1, 6, 6, 8, 0, 0, 0, 0, 1, 5, 3, 4, 0, 0, 0, 0, 3, 2, 3, 4, 0, 0, 0, 0, 4, 6, 6, 6, 0, 0, 0, 0, 3, 4, 5, 2, 1, 1, 2, 3, 0, 0, 0, 0, 1, 2, 3, 2, 2, 8, 6, 9, 2, 8, 6, 7, 3, 10, 6, 8, 0, 0, 0, 0, 6, 8, 9, 5, 2, 3, 1, 0, 1, 2, 2, 2, 3, 10, 6, 6, 3, 2, 1, 2, 6, 16, 12, 15, 10, 9, 2, 4, 2, 7, 5, 5, 3, 2, 0, 1, 0, 2, 1, 3, 0, 0, 0, 0, 1, 1, 3, 3, 4, 10, 5, 3, 0, 0, 0, 0, 0, 0, 0, 0, 3, 2, 1, 0, 2, 3, 0, 1, 1, 3, 2, 2, 2, 3, 0, 1, 2, 3, 1, 1, 0, 0, 0, 0, 0, 2, 1, 3, 1, 2, 3, 2, 0, 2, 2, 2, 1, 17, 12, 15, 1, 5, 6, 3, 4, 5, 2, 2, 9, 13, 8, 7, 3, 2, 1, 1, 2, 6, 4, 3, 0, 0, 0, 0, 0, 0, 0, 0, 1, 2, 1, 2, 0, 0, 0, 0, 0, 0, 0, 0, 0, 3, 2, 3, 1, 2, 1, 2, 4, 7, 6, 8, 5, 12, 9, 7, 0, 4, 5, 3, 2, 2, 1, 2, 5, 9, 5, 5, 4, 8, 6, 8, 3, 2, 1, 1, 0, 5, 4, 5, 4, 4, 2, 2, 3, 2, 2, 0, 3, 8, 6, 7, 3, 7, 4, 6, 0, 0, 0, 0, 0, 0, 0, 0, 1, 1, 2, 2, 0, 0, 0, 0, 1, 3, 2, 1, 0, 0, 0, 0, 0, 0, 0, 0, 0, 0, 0, 0, 0, 0, 0, 0, 0, 0, 0, 0, 0, 0, 0, 0, 0, 0, 0, 0, 0, 0, 0, 0, 2, 2, 1, 1, 2, 2, 1, 1, 1, 2, 1, 3, 0, 0, 0, 0, 0, 2, 3, 2, 2, 10, 9, 7, 3, 5, 3, 3, 1, 3, 4, 4, 0, 0, 0, 0, 0, 2, 3, 1, 0, 2, 3, 2, 0, 2, 3, 2, 0, 0, 0, 0, 3, 2, 2, 0, 3, 2, 2, 0, 0, 2, 2, 2, 0, 0, 0, 0, 1, 2, 1, 3], "Di_MxRight#"=[0, 0, 0, 0, 0, 0, 0, 0, 0, 0, 0, 0, 0, 0, 0, 0, 0, 0, 0, 0, 0, 0, 0, 0, 0, 0, 0, 0, 0, 0, 0, 0, 0, 0, 0, 0, 0, 0, 0, 0, 0, 0, 0, 0, 0, 0, 0, 0, 0, 0, 0, 0, 0, 0, 0, 0, 0, 0, 0, 0, 0, 0, 0, 0, 0, 0, 0, 0, 0, 0, 0, 0, 0, 2, 0, 1, 0, 0, 0, 1, 0, 1, 0, 0, 0, 2, 0, 1, 0, 0, 0, 1, 0, 1, 0, 0, 0, 0, 2, 0, 0, 1, 0, 0, 0, 1, 1, 1, 0, 0, 0, 0, 0, 0, 0, 0, 0, 0, 0, 0, 2, 0, 0, 1, 0, 1, 0, 0, 0, 1, 1, 0, 6, 2, 2, 2, 0, 3, 1, 0, 1, 4, 3, 0, 1, 2, 1, 1, 0, 1, 1, 1, 1, 2, 0, 1, 2, 0, 1, 1, 1, 1, 0, 1, 0, 2, 1, 0, 0, 0, 0, 0, 0, 0, 0, 0, 0, 0, 0, 0, 2, 0, 0, 1, 0, 1, 0, 0, 0, 0, 1, 0, 2, 0, 0, 1, 0, 1, 0, 0, 0, 1, 1, 0, 2, 0, 0, 1, 0, 1, 0, 0, 0, 1, 1, 0, 0, 0, 0, 0, 0, 0, 0, 0, 0, 0, 0, 0, 0, 2, 0, 1, 1, 0, 1, 1, 0, 0, 0, 0, 0, 2, 0, 1, 1, 0, 1, 1, 0, 0, 0, 0, 2, 0, 0, 0, 0, 2, 0, 0, 0, 1, 0, 0, 0, 0, 0, 0, 0, 0, 0, 0, 0, 0, 0, 0, 0, 0, 1, 0, 0, 1, 1, 0, 0, 1, 1, 1, 0, 0, 0, 0, 0, 0, 0, 0, 0, 0, 0, 0, 0, 0, 1, 0, 0, 0, 2, 0, 0, 0, 0, 2, 2, 0, 3, 1, 0, 3, 1, 0, 0, 2, 3, 1, 0, 0, 0, 0, 0, 0, 0, 0, 0, 0, 0, 0, 2, 0, 5, 1, 1, 4, 1, 0, 0, 3, 4, 0, 2, 1, 3, 2, 0, 2, 1, 0, 0, 3, 2, 0, 4, 0, 0, 1, 0, 3, 0, 0, 0, 2, 0, 0, 2, 0, 0, 1, 0, 1, 0, 0, 0, 1, 0, 0, 0, 0, 0, 0, 0, 0, 0, 0, 0, 0, 0, 0, 4, 0, 0, 1, 0, 3, 0, 0, 0, 2, 1, 0, 2, 0, 2, 0, 0, 3, 0, 0, 0, 3, 1, 0, 4, 0, 0, 1, 0, 3, 0, 0, 0, 3, 0, 0, 0, 0, 0, 0, 0, 0, 0, 0, 0, 0, 0, 0, 1, 0, 0, 1, 1, 1, 0, 0, 0, 0, 1, 0, 6, 0, 2, 1, 0, 6, 0, 0, 0, 4, 1, 0, 1, 0, 5, 0, 1, 2, 1, 0, 0, 3, 2, 0, 0, 0, 2, 1, 1, 1, 2, 0, 1, 0, 2, 1, 2, 2, 1, 1, 0, 2, 1, 1, 0, 3, 0, 0, 4, 0, 0, 2, 0, 2, 0, 0, 0, 1, 1, 0, 0, 0, 0, 0, 0, 0, 0, 0, 0, 0, 0, 0, 0, 3, 1, 0, 0, 0, 3, 0, 1, 1, 0, 1, 0, 0, 1, 0, 1, 1, 1, 0, 0, 0, 1, 0, 0, 2, 1, 1, 0, 0, 1, 1, 0, 1, 0, 0, 0, 0, 0, 0, 0, 0, 0, 0, 0, 0, 0, 0, 0, 0, 0, 0, 0, 0, 0, 0, 0, 0, 0, 0, 4, 1, 5, 1, 0, 5, 1, 0, 1, 5, 4, 2, 0, 0, 2, 0, 1, 0, 0, 0, 0, 1, 1, 0, 1, 1, 3, 0, 0, 2, 2, 0, 1, 3, 1, 1, 1, 0, 3, 0, 0, 2, 0, 0, 0, 3, 1, 0, 0, 1, 1, 1, 0, 0, 1, 0, 0, 1, 0, 0, 14, 0, 1, 5, 0, 8, 0, 0, 0, 6, 3, 0, 2, 0, 0, 1, 0, 1, 0, 0, 0, 0, 1, 0, 2, 0, 0, 1, 0, 1, 0, 0, 0, 0, 1, 0, 0, 0, 0, 0, 0, 0, 0, 0, 0, 0, 0, 0, 2, 1, 1, 2, 0, 1, 1, 1, 0, 1, 1, 0, 0, 0, 0, 0, 0, 0, 0, 0, 0, 0, 0, 0, 2, 0, 0, 0, 0, 2, 0, 0, 0, 1, 0, 0, 2, 1, 4, 2, 1, 1, 2, 0, 0, 2, 1, 1, 5, 3, 5, 3, 0, 3, 2, 1, 0, 6, 1, 0, 0, 0, 0, 0, 0, 0, 0, 0, 0, 0, 0, 0, 0, 0, 3, 1, 2, 1, 1, 2, 1, 2, 3, 0, 0, 0, 0, 0, 0, 0, 0, 0, 0, 0, 0, 0, 4, 1, 2, 1, 0, 2, 1, 1, 0, 4, 0, 1, 3, 0, 3, 1, 1, 4, 1, 0, 0, 3, 2, 0, 0, 0, 0, 0, 0, 0, 0, 0, 0, 0, 0, 0, 1, 1, 3, 1, 0, 1, 1, 0, 0, 2, 1, 0, 0, 0, 0, 0, 0, 0, 0, 0, 0, 0, 0, 0, 0, 1, 1, 0, 0, 2, 0, 1, 1, 1, 1, 2, 0, 0, 0, 0, 0, 0, 0, 0, 0, 0, 0, 0, 0, 2, 2, 3, 1, 2, 2, 1, 1, 1, 3, 1, 0, 0, 0, 0, 0, 0, 0, 0, 0, 0, 0, 0, 2, 2, 0, 2, 1, 1, 1, 1, 0, 1, 1, 0, 0, 0, 1, 0, 1, 1, 0, 1, 0, 1, 1, 0, 0, 0, 0, 0, 0, 0, 0, 0, 0, 0, 0, 0, 0, 0, 1, 1, 1, 1, 0, 1, 0, 0, 2, 0, 4, 1, 3, 0, 0, 4, 1, 0, 1, 5, 2, 0, 3, 2, 3, 2, 0, 3, 1, 1, 0, 3, 2, 0, 2, 2, 4, 2, 0, 3, 2, 1, 0, 3, 3, 1, 0, 0, 0, 0, 0, 0, 0, 0, 0, 0, 0, 0, 3, 2, 2, 3, 3, 2, 3, 2, 0, 0, 3, 1, 0, 2, 0, 1, 0, 0, 1, 1, 0, 0, 0, 0, 1, 0, 1, 1, 0, 0, 1, 0, 0, 0, 1, 1, 4, 2, 2, 2, 0, 3, 2, 1, 0, 3, 1, 1, 0, 1, 1, 0, 0, 0, 2, 0, 1, 0, 1, 1, 8, 4, 3, 2, 1, 8, 3, 1, 1, 9, 2, 0, 1, 5, 0, 0, 1, 0, 6, 0, 4, 2, 1, 1, 2, 2, 2, 2, 0, 2, 1, 1, 0, 2, 2, 0, 0, 1, 0, 0, 0, 0, 2, 0, 1, 0, 0, 1, 0, 0, 2, 0, 0, 1, 0, 0, 0, 1, 1, 0, 0, 0, 0, 0, 0, 0, 0, 0, 0, 0, 0, 0, 0, 0, 1, 0, 1, 1, 0, 1, 0, 1, 2, 0, 3, 4, 1, 3, 0, 1, 2, 1, 1, 3, 0, 0, 0, 0, 0, 0, 0, 0, 0, 0, 0, 0, 0, 0, 0, 0, 0, 0, 0, 0, 0, 0, 0, 0, 0, 0, 0, 2, 0, 1, 0, 0, 1, 1, 0, 0, 0, 0, 0, 2, 0, 0, 0, 0, 1, 0, 1, 1, 0, 0, 1, 1, 1, 1, 0, 1, 1, 0, 0, 1, 0, 0, 0, 2, 0, 0, 0, 0, 1, 0, 1, 1, 0, 0, 0, 2, 1, 1, 0, 0, 1, 1, 0, 0, 0, 0, 0, 0, 0, 0, 0, 0, 0, 0, 0, 0, 0, 0, 0, 0, 2, 0, 0, 1, 0, 0, 0, 1, 1, 0, 0, 0, 1, 1, 1, 1, 0, 1, 0, 0, 2, 0, 2, 0, 0, 0, 0, 1, 0, 0, 0, 2, 0, 0, 11, 1, 4, 2, 0, 7, 0, 0, 1, 11, 1, 0, 4, 0, 0, 2, 1, 2, 1, 0, 0, 1, 2, 0, 2, 2, 1, 0, 1, 0, 2, 0, 1, 1, 0, 1, 3, 4, 3, 3, 2, 2, 6, 3, 0, 2, 0, 3, 0, 2, 0, 1, 0, 0, 1, 1, 1, 0, 0, 0, 4, 1, 1, 1, 0, 1, 1, 0, 1, 3, 0, 0, 0, 0, 0, 0, 0, 0, 0, 0, 0, 0, 0, 0, 0, 0, 0, 0, 0, 0, 0, 0, 0, 0, 0, 0, 1, 0, 1, 0, 1, 0, 1, 0, 0, 1, 0, 0, 0, 0, 0, 0, 0, 0, 0, 0, 0, 0, 0, 0, 0, 0, 0, 0, 0, 0, 0, 0, 0, 0, 0, 0, 2, 0, 1, 0, 0, 2, 0, 0, 0, 2, 0, 0, 0, 0, 2, 0, 0, 0, 1, 0, 0, 1, 1, 0, 3, 2, 2, 0, 0, 3, 1, 1, 2, 4, 1, 2, 4, 2, 3, 3, 2, 3, 2, 2, 1, 4, 2, 0, 4, 0, 0, 2, 0, 2, 0, 0, 0, 1, 1, 0, 0, 0, 1, 0, 0, 1, 2, 0, 0, 0, 0, 2, 4, 2, 2, 2, 1, 0, 2, 0, 3, 3, 1, 1, 4, 1, 3, 1, 1, 2, 2, 0, 1, 4, 2, 1, 1, 1, 0, 0, 0, 0, 2, 0, 1, 0, 0, 1, 4, 0, 1, 0, 0, 3, 0, 0, 0, 4, 0, 0, 0, 4, 0, 2, 0, 0, 2, 0, 2, 0, 0, 0, 1, 1, 0, 1, 1, 0, 1, 1, 0, 0, 0, 0, 3, 1, 3, 2, 0, 3, 1, 1, 1, 4, 2, 0, 2, 2, 3, 2, 0, 2, 1, 1, 1, 2, 1, 0, 0, 0, 0, 0, 0, 0, 0, 0, 0, 0, 0, 0, 0, 0, 0, 0, 0, 0, 0, 0, 0, 0, 0, 0, 0, 0, 1, 1, 0, 1, 0, 0, 0, 0, 1, 1, 0, 0, 0, 0, 0, 0, 0, 0, 0, 0, 0, 0, 1, 1, 1, 1, 0, 0, 1, 0, 0, 1, 0, 0, 0, 0, 0, 0, 0, 0, 0, 0, 0, 0, 0, 0, 0, 0, 0, 0, 0, 0, 0, 0, 0, 0, 0, 0, 0, 0, 0, 0, 0, 0, 0, 0, 0, 0, 0, 0, 0, 0, 0, 0, 0, 0, 0, 0, 0, 0, 0, 0, 0, 0, 0, 0, 0, 0, 0, 0, 0, 0, 0, 0, 0, 0, 0, 0, 0, 0, 0, 0, 0, 0, 0, 0, 0, 0, 0, 0, 0, 0, 0, 0, 0, 0, 0, 0, 0, 0, 0, 0, 0, 0, 0, 0, 0, 0, 0, 0, 0, 2, 0, 1, 0, 0, 0, 1, 0, 1, 0, 0, 0, 2, 0, 1, 0, 0, 0, 1, 0, 1, 0, 0, 0, 0, 2, 0, 0, 1, 0, 0, 0, 1, 1, 1, 0, 0, 0, 0, 0, 0, 0, 0, 0, 0, 0, 0, 2, 0, 0, 1, 0, 1, 0, 0, 0, 1, 1, 0, 6, 2, 2, 2, 0, 3, 1, 0, 1, 4, 3, 0, 1, 2, 1, 1, 0, 1, 1, 1, 1, 2, 0, 1, 2, 0, 1, 1, 1, 1, 0, 1, 0, 2, 1, 0, 0, 0, 0, 0, 0, 0, 0, 0, 0, 0, 0, 0, 2, 0, 0, 1, 0, 1, 0, 0, 0, 0, 1, 0, 2, 0, 0, 1, 0, 1, 0, 0, 0, 1, 1, 0, 2, 0, 0, 1, 0, 1, 0, 0, 0, 1, 1, 0, 0, 0, 0, 0, 0, 0, 0, 0, 0, 0, 0, 0, 0, 2, 0, 1, 1, 0, 1, 1, 0, 0, 0, 0, 0, 2, 0, 1, 1, 0, 1, 1, 0, 0, 0, 0, 2, 0, 0, 0, 0, 2, 0, 0, 0, 1, 0, 0, 0, 0, 0, 0, 0, 0, 0, 0, 0, 0, 0, 0, 0, 0, 1, 0, 0, 1, 1, 0, 0, 1, 1, 1], "Mono_MxRight#"=array[5868 elements]} ("LSP_C2")
  w118 = -2532 ("specific error code to clear (0: all)")
  w292 = picture data[5B] ("All Radar_X")
  w295 = T26 {"X Values"=[], "Histogram: h(x)"=[]} ("Q_Histogram")
  w296 = string[] ["N_sort_B", "N_sort_[%]", "N_sort_#", "P_sort_B", "P_sort_[%]", "P_sort_#"] ("Column Header Strings[]")
  w299 = dbl[][] [] ("Total NGraph")
  w300 = string[][] [] ("Long Signal Profile Table")
  w293 = 0.0 ("coverage [%]")
  w294 = 0 ("S#")
  w268 = string[] [] ("Assigned_Array")
  w306 = i32[] [] ("appended array")
  w421 = 0 ("Assembly Ratio")
  w399 = 0.0 ("Assembly Ratio")
  w445 = "AC Table" ("グループ名入力")
  w450 = "R Table" ("グループ名入力")
  w402 = -10.0 ("カーソル.カーソル位置:カーソルX")
  w401 = -10.0 ("カーソル.カーソル位置:カーソルX")
  w325 = string[][] []
  w386 = 0
  w490 = "Table Tag" ("グループ名入力")
  w382 = string[][] []
  w488 = "B Table" ("グループ名入力")
  # "Data 消去 20221101"
  # "Ladar Array SAVE"
  # "MS_Plot Array SAVE"
  # "Signal# Histogram"
  # "QT Histogram Plot"
  # "BNAL Path Formation"
  # "BNAL Plot"
  # "BNAL Rader"
  # "Plot Array SAVE"
  # "BC Table"
  # "BR Table for TDMS"
  # "B Region Selection"
  # "ANAL info Extraction"
  # "B Region Read"
  # "Raw data Read (from ANAL)"
  n1 = property on="Q_Histogram" class="XYGraph (strict)"("Value"=w295) -> ()  [unwired: 2 in, 2 out]
  n2 = property on="Time Histogram" class="XYGraph (strict)"("Value"=w295) -> ()  [unwired: 2 in, 2 out]
  n3 = property on="Numeric" class="DigNum (strict)"(error in="error in", "Value"=4 ("Numeric")) -> (error out=w1:errorcluster)  [unwired: 1 in, 1 out]
  n4 = case shown="True" TRUE {
    tunnel: [w498 w501] -> w17
    tunnel: "S New Info and MiN" -> [w498 w503]
    tunnel: w1 -> [w499 w500]
    tunnel: [w499 w500] -> w15
    frame False {
    }
    frame True {
      n5 = call "Max_rr_base change.vi"("Numeric"="Numeric", "S New Info and MiN"=w503) -> ("S New Info and MiN 2"=w501:T28)  [unwired: 9 in]
    }
  }
  n6 = property on="Av RRn# kbp/day" class="DigNum (strict)"("Value"=w293) -> ()  [unwired: 2 in, 2 out]
  n7 = property on="Total AGraph" class="IntGraph (strict)"("Value"=w299) -> ()  [unwired: 2 in, 2 out]
  n8 = property on="Plot Graph" class="IntGraph (strict)"("Value"=w299) -> ()  [unwired: 2 in, 2 out]
  n9 = property on="Total NGraph" class="IntGraph (strict)"("Value"=w299) -> ()  [unwired: 2 in, 2 out]
  n10 = property on="Av n# kbp/day" class="DigNum (strict)"("Value"=w293) -> ()  [unwired: 2 in, 2 out]
  n11 = property on="coverage [%]" class="DigNum (strict)"("Value"=w293) -> ()  [unwired: 2 in, 2 out]
  n12 = property on="Av N_Read N" class="DigNum (strict)"("Value"=w293) -> ()  [unwired: 2 in, 2 out]
  n13 = property on="5’→3'" class="DigNum (strict)"("Value"=w293) -> ()  [unwired: 2 in, 2 out]
  n14 = property on="Av R_Read N" class="DigNum (strict)"("Value"=w293) -> ()  [unwired: 2 in, 2 out]
  n15 = call <vilib>:"Clear Errors.vi"("error in (no error)"=w15) -> ("error out"=w305:errorcluster)  [unwired: 5 in, 1 out]
  n16 = while {
    tunnel: w305 -> [w505]
    tunnel: [w505] -> w304
    i -> [w507]
    stop <- w508 stop-if-true
    n17 = local write "Control_2"(T22."Plot" ("Control_2")) -> ()
    n18 = Equal?(x=0, y=w507) -> (x = y?=w508:bool)
  }
  n19 = property on="Count Graph" class="XYGraph (strict)"("Value"=cluster{i32[], i32[]} {[], []} ("Count Graph")) -> ()  [unwired: 2 in, 2 out]
  n20 = property on="Signal# Histogram" class="XYGraph (strict)"("Value"=cluster{"配列 2":i32[], "配列 5":dbl[]}[] [] ("Signal Number Histogram")) -> ()  [unwired: 2 in, 2 out]
  n21 = property on="Mono Table" class="Tbl (strict)"("Value"=w300) -> ()  [unwired: 2 in, 2 out]
  n22 = property on="Tri Table" class="Tbl (strict)"("Value"=w300) -> ()  [unwired: 2 in, 2 out]
  n23 = property on="Di Table" class="Tbl (strict)"("Value"=w300) -> ()  [unwired: 2 in, 2 out]
  n24 = property on="Di Table" class="Tbl (strict)"("Column Headers[]"=w296) -> ()  [unwired: 2 in, 2 out]
  n25 = property on="Tri Table" class="Tbl (strict)"("Column Headers[]"=w296) -> ()  [unwired: 2 in, 2 out]
  n26 = property on="Covered?" class="Bool (strict)"("Value"=FALSE ("Covered?")) -> ()  [unwired: 2 in, 2 out]
  n27 = property on="Total BC" class="Arr (strict)"("Value"=bool[] [] ("Total BC")) -> ()  [unwired: 2 in, 2 out]
  n28 = property on="Long Assembly" class="Arr (strict)"("Value"=bool[][] [] ("Long Assembly")) -> ()  [unwired: 2 in, 2 out]
  n29 = property on="Mono Table" class="Tbl (strict)"("Column Headers[]"=w296) -> ()  [unwired: 2 in, 2 out]
  n30 = property on="S New Info and MiN" class="Clust (strict)"(error in=w304, "Value"=w17) -> (error out=w405:errorcluster)  [unwired: 1 in, 1 out]
  n31 = property on="S New Info and MiN" class="Clust (strict)"(error in=w405) -> (error out=w197:errorcluster, "Value"=w397:T28)  [unwired: 1 in, 1 out]
  n32 = property on="RR#" class="DigNum (strict)"("Value"=w294) -> ()  [unwired: 2 in, 2 out]
  n33 = property on="S#" class="DigNum (strict)"("Value"=w294) -> ()  [unwired: 2 in, 2 out]
  n34 = property on="MAX RR#" class="DigNum (strict)"("Value"=w294) -> ()  [unwired: 2 in, 2 out]
  n35 = property on="All Radar_X" class="Pict"("Value"=w292) -> ()  [unwired: 2 in, 2 out]
  n36 = property on="All Radar Plot_XX" class="Pict"("Value"=w292) -> ()  [unwired: 2 in, 2 out]
  n37 = property on="Total Base CP" class="DigNum (strict)"("Value"=w294) -> ()  [unwired: 2 in, 2 out]
  n38 = property on="RR MIN Over S#" class="DigNum (strict)"("Value"=w294) -> ()  [unwired: 2 in, 2 out]
  n39 = property on="Av RR n#bp" class="DigNum (strict)"("Value"=w294) -> ()  [unwired: 2 in, 2 out]
  n40 = property on="B_Region#" class="DigNum (strict)"("Value"=w294) -> ()  [unwired: 2 in, 2 out]
  n41 = property on="Av n#bp" class="DigNum (strict)"("Value"=w294) -> ()  [unwired: 2 in, 2 out]
  n42 = case shown="False" "Locked" {
    tunnel: w197 -> [w512 w517]
    tunnel: w397 -> [w515 w516]
    tunnel: [w509 w517] -> w34
    tunnel: [w513 w516] -> w196
    frame False {
      n43 = call "test panel for 2nd.vi"("error in"=w512, "S New Info and MiN"=w515) -> ("error out"=w514:errorcluster, "S New Info and MiN out"=w513:T28)  [unwired: 7 in, 1 out]
      n44 = property on="S New Info and MiN" class="Clust (strict)"(error in=w514, "Value"=w513) -> (error out=w510:errorcluster)  [unwired: 1 in, 1 out]
      n45 = property on="Locked" class="Bool (strict)"(error in=w510, "Value"=TRUE ("Locked")) -> (error out=w509:errorcluster)  [unwired: 1 in, 1 out]
    }
    frame True {
    }
  }
  n46 = property on="LCP_C1" class="Clust (strict)"("Value"=cluster{dbl[], dbl[], i32[], dbl[]} {[], [], [], []} ("LCP_C1")) -> ()  [unwired: 2 in, 2 out]
  n47 = property on="AR#" class="Arr (strict)"("Value"=w306) -> ()  [unwired: 2 in, 2 out]
  n48 = property on="RR#" class="Arr (strict)"("Value"=w306) -> ()  [unwired: 2 in, 2 out]
  n49 = Unbundle(w196) -> ("Sample Sequence"=w398:string, "Right Read MIN"=w307:i32, "Base Table"=w335:T32, "noise MAX"=w317:i32)  [unwired: 4 out]
  n50 = call "ASM MIni Stat.vi"("error in"=w34, "Base Table"=w335, "Sample Sequence"=w398, "Right Read MIN"=w307) -> ("SB_ANA"=w209:T25, "error out"=w33:errorcluster)  [unwired: 5 in, 1 out]
  n51 = call "ASD Base info.vi"("Base Table"=w335) -> ("Base N info"=w321:T33)  [unwired: 8 in, 2 out]
  n52 = Unbundle(w321) -> ("Base Composition"=w313:string[], "Base S Level"=w320:dbl[], "Color IDX"=w314:u32[])  [unwired: 3 out]
  n53 = call "ASD Color Label.vi"("Level Composition"=w313, "Color"=w314) -> ("Label"=→"Label" →"Label 2" →"Label 3":T23)  [unwired: 9 in]
  n54 = property on="S New Info and MiN" class="Clust (strict)"(error in=w33, "Value"=w196) -> (error out=w328:errorcluster)  [unwired: 1 in, 1 out]
  n55 = property on="Level Composition" class="Arr (strict)"(error in=w328, "Value"=w313) -> (error out=w319:errorcluster)  [unwired: 1 in, 1 out]
  n56 = property on="Base R Level" class="Arr (strict)"(error in=w319, "Value"=w320) -> (error out=w318:errorcluster)  [unwired: 1 in, 1 out]
  n57 = property on="Base Color" class="Arr (strict)"(error in=w318, "Value"=w314) -> (error out=w316:errorcluster)  [unwired: 1 in, 1 out]
  n58 = property on="noise MAX" class="DigNum (strict)"(error in=w316, "Value"=w317) -> (error out=w208:errorcluster)  [unwired: 1 in, 1 out]
  n59 = property on="SB_ANA" class="Clust (strict)"(error in=w208, "Value"=w209) -> (error out=w207:errorcluster)  [unwired: 1 in, 1 out]
  n60 = Get Date/Time In Seconds() -> (seconds since 1Jan1904=w424:timestamp)
  n61 = property on="S New Info and MiN" class="Clust (strict)"(error in=w207) -> (error out=w406:errorcluster, "Value"=w407:T28)  [unwired: 1 in, 1 out]
  n62 = Format Date/Time String(time format string (%c)="@%Y_%m%d_%H%M" ("時間形式文字列（%c）"), seconds (now)=w424) -> (date/time string=w263:string)  [unwired: 1 in]
  n63 = Format Date/Time String(time format string (%c)="%d:%H:%M:%S" ("時間形式文字列（%c）"), seconds (now)=w424) -> (date/time string=w422:string)  [unwired: 1 in]
  n64 = Unbundle(w407) -> ("Sample Sequence"=w67:string, "Right Read MIN"=w409:i32, "Base Table"=w415:T32, "Selection"=w418:enum16{"10kHz", "100kHz"}, "noise MAX"=w411:i32, "Sample name"=w259:string)  [unwired: 2 out]
  n65 = Array Size(array=w415) -> (size(s)=w414:i32)
  n66 = call "Each Base Sequence Analysis.vi"("Sample Sequence"=w67) -> ("Cutted Sequence"=w413:string, "Base (n)"=w416:i32)  [unwired: 7 in, 2 out]
  n67 = Bundle("Assembly Ratio"=w399, "Assembly Ratio"=w421, "Assembly Ratio"=w421, "Assembly Ratio"=w399) -> (w420:T34)  [unwired: 1 in]
  n68 = property on="B Table" class="Tbl (strict)"(error in=w406, "Value"=w325) -> (error out=w474:errorcluster)  [unwired: 1 in, 1 out]
  n69 = property on="Right Read MIN" class="DigNum (strict)"(error in=w474, "Value"=w409) -> (error out=w473:errorcluster)  [unwired: 1 in, 1 out]
  n70 = property on="Base (n)" class="DigNum (strict)"(error in=w473, "Value"=w416) -> (error out=w472:errorcluster)  [unwired: 1 in, 1 out]
  n71 = property on="Base Species (n)" class="DigNum (strict)"(error in=w472, "Value"=w414) -> (error out=w471:errorcluster)  [unwired: 1 in, 1 out]
  n72 = property on="Cutted Sample Sequence" class="Str"(error in=w471, "Value"=w413) -> (error out=w463:errorcluster)  [unwired: 1 in, 1 out]
  n73 = property on="Date" class="Str"(error in=w463, "Value"=w263) -> (error out=w323:errorcluster)  [unwired: 1 in, 1 out]
  n74 = property on="BS Table" class="Tbl (strict)"(error in=w323, "Value"=w325) -> (error out=w423:errorcluster)  [unwired: 1 in, 1 out]
  n75 = property on="before" class="Str"(error in=w423, "Value"=w422) -> (error out=w419:errorcluster)  [unwired: 1 in, 1 out]
  n76 = property on="Total assembly C" class="Clust (strict)"(error in=w419, "Value"=w420) -> (error out=w412:errorcluster)  [unwired: 1 in, 1 out]
  n77 = property on="Selection" class="Enum (strict)"(error in=w412, "Value"=w418) -> (error out=w410:errorcluster)  [unwired: 1 in, 1 out]
  n78 = property on="noise MAX" class="DigNum (strict)"(error in=w410, "Value"=w411) -> (error out=w327:errorcluster)  [unwired: 1 in, 1 out]
  n79 = property on="LSP Table" class="Tbl (strict)"(error in=w327, "Value"=w325) -> (error out=w326:errorcluster)  [unwired: 1 in, 1 out]
  n80 = property on="LCP Table" class="Tbl (strict)"(error in=w326, "Value"=w325) -> (error out=w66:errorcluster)  [unwired: 1 in, 1 out]
  n81 = property on="Sample Sequence" class="Str"(error in=w66, "Value"=w67) -> (error out=w65:errorcluster)  [unwired: 1 in, 1 out]
  n82 = Concatenate Strings("@" ("string"), w259) -> (w260:string)
  n83 = call "BSD_Filename Path formation_MS.vi"("BF_name"=w260, "error in (no error)"=w65, "Date"=w263, "SAVE"=FALSE, "Filename Path"="Filename") -> ("error out"=w261:errorcluster, "BNAL Path"=w262:T16, "FN#"=w19:string)  [unwired: 2 in, 2 out]
  n84 = property on="BNAL Path" class="Clust (strict)"(error in=w261, "Value"=w262) -> (error out=w395:errorcluster)  [unwired: 1 in, 1 out]
  n85 = property on="BNAL Path" class="Clust (strict)"(error in=w395) -> (error out=w391:errorcluster, "Value"=w462:T16)  [unwired: 1 in, 1 out]
  n86 = property on="Selection" class="Enum (strict)"(error in=w391) -> (error out=w21:errorcluster, "Value"=w417:enum16{"10kHz", "100kHz"})  [unwired: 1 in, 1 out]
  n87 = property on="FN#" class="Str"(error in=w21, "Value"=w19) -> (error out=w20:errorcluster)  [unwired: 1 in, 1 out]
  n88 = case shown="\"10kHz\", Default" w417 {
    tunnel: [10000 ("R B_SCount [n] in") 100000 ("R B_SCount [n] in")] -> w429
    frame "10kHz", Default {
    }
    frame "100kHz" {
    }
  }
  "1s datapoint" <- w429
  n89 = Unbundle(w462) -> ("B_TDMS Path"=w394:string, "B_Folder Path"=w461:string)  [unwired: 4 out]
  n90 = String To Path(string=w394) -> (path=w393:path)
  n91 = property on="B_TDMS_Path" class="Path"(error in=w20, "Value"=w393) -> (error out=w392:errorcluster)  [unwired: 1 in, 1 out]
  n92 = property on="Folder Path" class="Str"(error in=w392, "Value"=w461) -> (error out=w334:errorcluster)  [unwired: 1 in, 1 out]
  n93 = property on="Folder Path" class="Str"(error in=w334) -> (error out=w333:errorcluster, "Value"=w291:string)  [unwired: 1 in, 1 out]
  n94 = property on="Right Read MIN" class="DigNum (strict)"(error in=w333) -> (error out=w332:errorcluster, "Value"=w288:i32)  [unwired: 1 in, 1 out]
  n95 = property on="Date" class="Str"(error in=w332) -> (error out=w331:errorcluster, "Value"=w290:string)  [unwired: 1 in, 1 out]
  n96 = property on="Level Composition" class="Arr (strict)"(error in=w331) -> (error out=w275:errorcluster, "Value"=w289:string[])  [unwired: 1 in, 1 out]
  n97 = call "BNAL Intial txt and tdms tag_MS.vi"("error in (no error)"=w275, "Level Composition"=w289, "Date"=w290, "Right Read MIN"=w288, "Folder Path"=w291) -> ("L_Tag cluster"=w267:T7, "CSV_Path cluster"=w287:T35, "error out"=w274:errorcluster)  [unwired: 3 in, 1 out]
  n98 = Unbundle(w287) -> ("LSP Table Pass"=w286:path, "LCP Table Pass"=w285:path, "LTP Table Pass"=w284:path)
  n99 = Unbundle(w267) -> ("LSP Table Tag"=w280:string[], "LCP Table Tag"=w279:string[], "LTP Table Tag"=w278:string[], "BS Table Tag"=w281:string[])  [unwired: 1 out]
  n100 = property on="LSP Table Pass" class="Path"(error in=w274, "Value"=w286) -> (error out=w330:errorcluster)  [unwired: 1 in, 1 out]
  n101 = property on="LCP Table Pass" class="Path"(error in=w330, "Value"=w285) -> (error out=w283:errorcluster)  [unwired: 1 in, 1 out]
  n102 = property on="LTP Table Pass" class="Path"(error in=w283, "Value"=w284) -> (error out=w282:errorcluster)  [unwired: 1 in, 1 out]
  n103 = property on="LSP Table Tag" class="Arr (strict)"(error in=w282, "Value"=w280) -> (error out=w329:errorcluster)  [unwired: 1 in, 1 out]
  n104 = property on="LCP Table Tag" class="Arr (strict)"(error in=w329, "Value"=w279) -> (error out=w277:errorcluster)  [unwired: 1 in, 1 out]
  n105 = property on="LTP Table Tag" class="Arr (strict)"(error in=w277, "Value"=w278) -> (error out=w276:errorcluster)  [unwired: 1 in, 1 out]
  n106 = property on="BS Table Tag" class="Arr (strict)"(error in=w276, "Value"=w281) -> (error out=w322:errorcluster)  [unwired: 1 in, 1 out]
  n107 = property on="BS Table" class="Tbl (strict)"(error in=w322, "Column Headers[]"=w281) -> (error out=w266:errorcluster)  [unwired: 1 in, 1 out]
  n108 = property on="Tag cluster_B" class="Clust (strict)"(error in=w266, "Value"=w267) -> (error out=w13:errorcluster)  [unwired: 1 in, 1 out]
  n109 = TDMS Open(8:w13, 10:T31."open" ("操作（0:open）"), 11:"Filename") -> (0:w12:errorcluster, 3:w496:refnum<k34>)  [unwired: 4 in]
  "error out 3" <- w12
  n110 = TDMS Read(0:w496, 5:"Data" ("グループ名入力（名称未設定）"), 11:w12, 12:dbl[] [] ("配列")) -> (4:w491:refnum<k34>, 10:→"Raw data" →"Raw data Graph":dbl[], 15:w492:errorcluster)  [unwired: 4 in, 3 out]
  n111 = TDMS Read(0:w491, 5:w490, 11:w492) -> (4:w447:refnum<k34>, 8:w434:string[], 15:w435:errorcluster)  [unwired: 5 in, 3 out]
  n112 = property on="Channel Tag" class="Arr (strict)"(error in=w435, "Value"=w434) -> (error out=w390:errorcluster)  [unwired: 1 in, 1 out]
  n113 = TDMS Read(0:w447, 5:w490, 11:w390, 12:string[][] []) -> (4:w381:refnum<k34>, 10:w439:string[][], 15:w438:errorcluster)  [unwired: 4 in, 3 out]
  n114 = property on="Table Tag" class="Arr (strict)"(error in=w438, "Value"=w439) -> (error out=w433:errorcluster)  [unwired: 1 in, 1 out]
  n115 = property on="Channel Tag" class="Arr (strict)"(error in=w433) -> (error out=w14:errorcluster, "Value"=w432:string[])  [unwired: 1 in, 1 out]
  n116 = Array Size(array=w432) -> (size(s)=w489:i32)
  n117 = for {
    N: w489 -> [_]
    tunnel: w432 -> [w524] mode=indexing
    tunnel: w488 -> [w541]
    shift-right: [w539] -> w487
    shift-left: w386 -> [w540]
    tunnel: w450 -> [w535]
    shift-right: [w537] -> w457
    shift-left: w386 -> [w536]
    shift-right: [w531] -> w453
    shift-left: w386 -> [w530]
    tunnel: w445 -> [w532]
    tunnel: "S Table" ("グループ名入力") -> [w529]
    shift-right: [w528] -> w388
    shift-left: w386 -> [w527]
    tunnel: "AR Table" ("グループ名入力") -> [w525]
    shift-right: [w523] -> w385
    shift-left: w386 -> [w522]
    i -> [w521]
    n118 = Equal?(x=w524, y=w529) -> (x = y?=w526:bool)
    n119 = Equal?(x=w524, y=w525) -> (x = y?=w520:bool)
    n120 = Equal?(x=w524, y=w535) -> (x = y?=w534:bool)
    n121 = Equal?(x=w524, y=w532) -> (x = y?=w533:bool)
    n122 = Equal?(x=w524, y=w541) -> (x = y?=w538:bool)
    n123 = case shown="True" w520 {
      tunnel: w521 -> [_ w543]
      tunnel: [w542 w543] -> w523
      tunnel: w522 -> [w542 _]
      frame False {
      }
      frame True {
      }
    }
    n124 = case shown="False" w526 {
      tunnel: w521 -> [_ w545]
      tunnel: [w544 w545] -> w528
      tunnel: w527 -> [w544 _]
      frame False {
      }
      frame True {
      }
    }
    n125 = case shown="False" w534 {
      tunnel: w521 -> [_ w549]
      tunnel: [w548 w549] -> w537
      tunnel: w536 -> [w548 _]
      frame False {
      }
      frame True {
      }
    }
    n126 = case shown="False" w533 {
      tunnel: w521 -> [_ w547]
      tunnel: [w546 w547] -> w531
      tunnel: w530 -> [w546 _]
      frame False {
      }
      frame True {
      }
    }
    n127 = case shown="False" w538 {
      tunnel: w521 -> [_ w551]
      tunnel: [w550 w551] -> w539
      tunnel: w540 -> [w550 _]
      frame False {
      }
      frame True {
      }
    }
  }
  n128 = property on="Table Tag" class="Arr (strict)"(error in=w14) -> (error out=w437:errorcluster, "Value"=w436:string[][])  [unwired: 1 in, 1 out]
  n129 = Index Array(array=w436, index (row) #1=w487, index (row) #2=w457, index (row) #3=w453, index (row) #4=w388, index (row) #5=w385) -> (element #1=w441:string[], element #2=w440:string[], element #3=w452:string[], element #4=→"S Table Tag":string[], element #5=→"AR Table Tag":string[])  [unwired: 5 in]
  "B Table Tag" <- w441
  "R Table Tag" <- w440
  "AC Table Tag" <- w452
  n130 = property on="B Table" class="Tbl (strict)"(error in=w437, "Column Headers[]"=w441) -> (error out=w456:errorcluster)  [unwired: 1 in, 1 out]
  n131 = property on="Assigned_Array" class="Arr (strict)"("Value"=w268) -> ()  [unwired: 2 in, 2 out]
  n132 = property on="MxRight_Array" class="Arr (strict)"("Value"=w268) -> ()  [unwired: 2 in, 2 out]
  n133 = property on="LSP_C2" class="Clust (strict)"("Value"=T8 {"Assigned Sequence"=[], "Mx Right Read Seq"=[]} ("LSP_C2")) -> ()  [unwired: 2 in, 2 out]
  n134 = property on="LSP_C1" class="Clust (strict)"("Value"=T9 {"Q value [x]"=[], "Signal Length [ms]"=[], "5’→3'"=[], "Seq SNo"=[], "Seq ENo"=[], "Mx Right No"=[]} ("LSP_C1")) -> ()  [unwired: 2 in, 2 out]
  n135 = property on="R Table" class="Tbl (strict)"(error in=w456, "Column Headers[]"=w440) -> (error out=w455:errorcluster)  [unwired: 1 in, 1 out]
  n136 = property on="AC Table" class="Tbl (strict)"(error in=w455, "Row Headers[]"=w452) -> (error out=w454:errorcluster)  [unwired: 1 in, 1 out]
  n137 = TDMS Read(0:w381, 5:w488, 11:w454, 12:w382) -> (4:w446:refnum<k34>, 10:w479:string[][], 15:w123:errorcluster)  [unwired: 4 in, 3 out]
  n138 = Transpose 2D Array(2D array=w479) -> (transposed array=w480:string[][])
  n139 = call <vilib>:"Clear Errors.vi"("error in (no error)"=w123, "specific error code to clear (0: all)"=w118) -> ("error out"=w120:errorcluster)  [unwired: 4 in, 1 out]
  n140 = Index Array(array=w479, index (row) #1=1 ("指標 （行）"), index (row) #2=2 ("指標 （行）")) -> (element #1=w484:string[], element #2=w483:string[])  [unwired: 2 in]
  n141 = property on="B Table" class="Tbl (strict)"(error in=w120, "Value"=w480) -> (error out=w451:errorcluster)  [unwired: 1 in, 1 out]
  n142 = Array Size(array=w480) -> (size(s)=w486:i32[])
  n143 = TDMS Read(0:w446, 5:w450, 11:w451, 12:w382) -> (4:w396:refnum<k34>, 10:w449:string[][], 15:w122:errorcluster)  [unwired: 4 in, 3 out]
  n144 = Fract/Exp String To Number(string=w484) -> (number=→"B Start [s]":dbl[])  [unwired: 3 in, 1 out]
  n145 = Fract/Exp String To Number(string=w483) -> (number=→"B End [s]":dbl[])  [unwired: 3 in, 1 out]
  n146 = Transpose 2D Array(2D array=w449) -> (transposed array=w448:string[][])
  n147 = call <vilib>:"Clear Errors.vi"("error in (no error)"=w122, "specific error code to clear (0: all)"=w118) -> ("error out"=w121:errorcluster)  [unwired: 4 in, 1 out]
  n148 = property on="R Table" class="Tbl (strict)"(error in=w121, "Value"=w448) -> (error out=w444:errorcluster)  [unwired: 1 in, 1 out]
  n149 = TDMS Read(0:w396, 5:w445, 11:w444, 12:w382) -> (10:w442:string[][], 15:w443:errorcluster)  [unwired: 4 in, 4 out]
  n150 = property on="AC Table" class="Tbl (strict)"(error in=w443, "Value"=w442) -> (error out=w119:errorcluster)  [unwired: 1 in, 1 out]
  n151 = call <vilib>:"Clear Errors.vi"("error in (no error)"=w119, "specific error code to clear (0: all)"=w118) -> ("error out"=w43:errorcluster)  [unwired: 4 in, 1 out]
  n152 = call "temp_test.vi"("error in (no error)"=w43) -> ("error out"=w42:errorcluster, "temp tdms_path B"=w41:path)  [unwired: 6 in, 3 out]
  n153 = Index Array(array=w486, index=0 ("指標")) -> (element=w475:i32)
  "Total B Region#" <- w475
  n154 = property on="B_TDMS_Path_Temp" class="Path"(error in=w42, "Value"=w41) -> (error out=w40:errorcluster)  [unwired: 1 in, 1 out]
  n155 = property on="B_TDMS_Path_Temp" class="Path"(error in=w40) -> (error out=w38:errorcluster, "Value"=w39:path)  [unwired: 1 in, 1 out]
  n156 = Copy(8:w38, 9:FALSE ("上書き（F）"), 10:w39, 11:"Filename") -> (0:w7:errorcluster, 3:w9:path)  [unwired: 1 in, 1 out]
  n157 = TDMS Delete Data(8:w7, 9:"Ch1" ("group name in"), 10:"Data" ("group name in"), 11:w9) -> (0:w6:errorcluster, 3:w8:path)  [unwired: 3 in]
  n158 = property on="S New Info and MiN" class="Clust (strict)"(error in=w6) -> (error out=w108:errorcluster, "Value"=w273:T28)  [unwired: 1 in, 1 out]
  n159 = property on="Tag cluster_B" class="Clust (strict)"(error in=w108) -> (error out=w107:errorcluster, "Value"=w109:T7)  [unwired: 1 in, 1 out]
  n160 = call "Bnal BC table VI_MS.vi"("error in"=w107, "S New Info and MiN"=w273, "Filename"=w8) -> ("error out"=w271:errorcluster, "TDMSファイル out"=w272:refnum<k34>)  [unwired: 7 in]
  n161 = call "BNAL Tdms opne intial_MS.vi"("error in"=w271, "Tag cluster_B"=w109, "TDMSファイル入力"=w272) -> ("error out"=w270:errorcluster, "A TDMSファイル出力"=w269:refnum<k34>)  [unwired: 7 in]
  n162 = property on="TDMS Tpath" class="Ref (strict)"(error in=w270, "Value"=w269) -> (error out=w265:errorcluster)  [unwired: 1 in, 1 out]
  n163 = property on="Time Graph" class="XYGraph (strict)"(error in=w265, "Active Cursor"=u32 4 ("アクティブカーソル"), "Cursor.Cursor Y"=w402, "Active Cursor"=u32 5 ("アクティブカーソル"), "Cursor.Cursor Y"=w402, "Active Cursor"=u32 6 ("アクティブカーソル"), "Cursor.Cursor Y"=w402) -> (error out=w458:errorcluster)  [unwired: 1 in, 1 out]
  n164 = property on="Data Histogram" class="XYGraph (strict)"(error in=w458, "Active Cursor"=u32 4 ("アクティブカーソル"), "Cursor.Cursor X"=w401, "Active Cursor"=u32 5 ("アクティブカーソル"), "Cursor.Cursor X"=w401, "Active Cursor"=u32 6 ("アクティブカーソル"), "Cursor.Cursor X"=w401) -> (error out=w310:errorcluster)  [unwired: 1 in, 1 out]
  n165 = property on="B Start [s]" class="Arr (strict)"(error in=w310) -> (error out=w309:errorcluster, "Value"=w312:dbl[])  [unwired: 1 in, 1 out]
  n166 = property on="B End [s]" class="Arr (strict)"(error in=w309) -> (error out=w308:errorcluster, "Value"=w311:dbl[])  [unwired: 1 in, 1 out]
  n167 = for {
    N: w475 -> [_]
    shift-right: [w646] -> w106
    shift-left: w308 -> [w709]
    tunnel: w312 -> [w661] mode=indexing
    tunnel: w311 -> [w659] mode=indexing
    tunnel: w475 -> [w726]
    i -> [w727]
    # "◎"
    # "◎"
    # "◎"
    # "B_Signal Total Numbering"
    # "Data Accumulation"
    # "Data Selection"
    # "Graph Formation"
    # "Burst Analysis"
    # "Signal Number extraction"
    # "BNAL TDMS SAVE"
    # "BNAL Time Count"
    # "10kHz"
    n168 = Increment(x=w727) -> (x+1=w681:i32)
    n169 = property on="B Table" class="Tbl (strict)"(error in=w709) -> (error out=w685:errorcluster, "Value"=w708:string[][])  [unwired: 1 in, 1 out]
    n170 = property on="B Table Tag" class="Arr (strict)"(error in=w685) -> (error out=w683:errorcluster, "Value"=w686:string[])  [unwired: 1 in, 1 out]
    n171 = property on="R Table Tag" class="Arr (strict)"(error in=w683) -> (error out=w682:errorcluster, "Value"=w684:string[])  [unwired: 1 in, 1 out]
    n172 = property on="R Table" class="Tbl (strict)"(error in=w682) -> (error out=w663:errorcluster, "Value"=w706:string[][])  [unwired: 1 in, 1 out]
    n173 = property on="B_Start [s]" class="DigNum (strict)"(error in=w663, "Value"=w661) -> (error out=w662:errorcluster)  [unwired: 1 in, 1 out]
    n174 = property on="B_END [s]" class="DigNum (strict)"(error in=w662, "Value"=w659) -> (error out=w603:errorcluster)  [unwired: 1 in, 1 out]
    n175 = Index Array(array=w708, index (row)=w681) -> (element=w707:string[])  [unwired: 1 in]
    "B info" <- w707
    n176 = Divide(x=w681, y=w726) -> (x/y=w729:dbl)
    n177 = call "BSD BR all info cluster.vi"("R Table"=w706, "R Table Tag"=w684, "B Table Tag"=w686, "B info"=w707) -> ("BR all info"=w657:T15)  [unwired: 7 in]
    n178 = Multiply(x=w729, y=100.0) -> (x*y=→"Progress":dbl)
    n179 = property on="B_Region#" class="DigNum (strict)"(error in=w603, "Value"=w681) -> (error out=w605:errorcluster)  [unwired: 1 in, 1 out]
    n180 = property on="Date" class="Str"(error in=w605) -> (error out=w604:errorcluster, "Value"=w710:string)  [unwired: 1 in, 1 out]
    n181 = property on="BR time [s]" class="DigNum (strict)"(error in=w604, "Value"=w659) -> (error out=w648:errorcluster)  [unwired: 1 in, 1 out]
    n182 = property on="BR all info" class="Clust (strict)"(error in=w648, "Value"=w657) -> (error out=w647:errorcluster)  [unwired: 1 in, 1 out]
    n183 = property on="Raw data" class="Arr (strict)"(error in=w647) -> (error out=w652:errorcluster, "Value"=w660:dbl[])  [unwired: 1 in, 1 out]
    n184 = property on="B_END [s]" class="DigNum (strict)"(error in=w652) -> (error out=w651:errorcluster, "Value"=w649:dbl)  [unwired: 1 in, 1 out]
    n185 = property on="B_Start [s]" class="DigNum (strict)"(error in=w651) -> (error out=w602:errorcluster, "Value"=w650:dbl)  [unwired: 1 in, 1 out]
    n186 = property on="1s datapoint" class="DigNum (strict)"(error in=w602) -> (error out=w601:errorcluster, "Value"=w654:i32)  [unwired: 1 in, 1 out]
    n187 = Bundle(w681, "Value"=w710) -> (w606:cluster{i32, "Value":string})  [unwired: 1 in]
    n188 = call "B_region_selection for ANAL.vi"("datapoint"=w654, "B_END [s]"=w649, "B_Start [s]"=w650, "Raw data"=w660) -> ("Selected Raw D"=w655:T21)  [unwired: 5 in, 2 out]
    n189 = property on="Raw data Graph" class="WFGraph (strict)"(error in=w601, "Active Cursor"=u32 0 ("アクティブカーソル"), "Cursor.Cursor X"=w659) -> (error out=w653:errorcluster)  [unwired: 1 in, 1 out]
    n190 = property on="Selected Raw D" class="Clust (strict)"(error in=w653, "Value"=w655) -> (error out=w600:errorcluster)  [unwired: 1 in, 1 out]
    n191 = property on="BC1" class="Clust (strict)"(error in=w600, "Value"=w606) -> (error out=w593:errorcluster)  [unwired: 1 in, 1 out]
    n192 = property on="BR all info" class="Clust (strict)"(error in=w593) -> (error out=w592:errorcluster, "Value"=w656:T15)  [unwired: 1 in, 1 out]
    n193 = property on="Total assembly C" class="Clust (strict)"(error in=w592) -> (error out=w607:errorcluster, "Value"=w674:T24)  [unwired: 1 in, 1 out]
    n194 = property on="Filename" class="Path"(error in=w607) -> (error out=w705:errorcluster, "Value"=w676:path)  [unwired: 1 in, 1 out]
    n195 = property on="S New Info and MiN" class="Clust (strict)"(error in=w705) -> (error out=w599:errorcluster, "Value"=w675:T28)  [unwired: 1 in, 1 out]
    n196 = property on="Selected Raw D" class="Clust (strict)"(error in=w599) -> (error out=w591:errorcluster, "Value"=w658:T21)  [unwired: 1 in, 1 out]
    n197 = property on="BC1" class="Clust (strict)"(error in=w591) -> (error out=w598:errorcluster, "Value"=w608:cluster{"B region#":i32, "Date":string})  [unwired: 1 in, 1 out]
    n198 = call "Base assingnment EXVI_MS.vi"("BR all info"=w656, "Total assembly C"=w674, "BC1"=w608, "error in"=w598, "Selected Raw D"=w658, "S New Info and MiN"=w675, "Filename Path"=w676) -> ("error out"=w578:errorcluster, "GR data"=w671:T20, "Data Histogram"=w672:T26, "Table cluster_B"=w579:T3, "Ex info"=w673:T36)
    n199 = Unbundle(w673) -> ("Base Ex Info"=w724:T18)  [unwired: 1 out]
    n200 = Unbundle(w579) -> ("LSP Table"=w670:string[][], "LCP Table"=w669:string[][], "LTP Table"=w668:string[][], "BS Table"=w667:string[][], "LAP Table"=w571:string[][])
    n201 = Unbundle(w724) -> ("Base A Level"=w723:dbl[])  [unwired: 6 out]
    n202 = property on="Table cluster_B" class="Clust (strict)"(error in=w578, "Value"=w579) -> (error out=w577:errorcluster)  [unwired: 1 in, 1 out]
    n203 = property on="LSP Table" class="Tbl (strict)"(error in=w577, "Value"=w670) -> (error out=w666:errorcluster)  [unwired: 1 in, 1 out]
    n204 = property on="LCP Table" class="Tbl (strict)"(error in=w666, "Value"=w669) -> (error out=w665:errorcluster)  [unwired: 1 in, 1 out]
    n205 = property on="LTP Table" class="Tbl (strict)"(error in=w665, "Value"=w668) -> (error out=w664:errorcluster)  [unwired: 1 in, 1 out]
    n206 = property on="BS Table" class="Tbl (strict)"(error in=w664, "Value"=w667) -> (error out=w573:errorcluster)  [unwired: 1 in, 1 out]
    n207 = property on="LAP Table" class="Tbl (strict)"(error in=w573, "Value"=w571) -> (error out=w572:errorcluster)  [unwired: 1 in, 1 out]
    n208 = property on="Data Histogram" class="XYGraph (strict)"(error in=w572, "Value"=w672) -> (error out=w711:errorcluster)  [unwired: 1 in, 1 out]
    n209 = property on="GR data" class="Clust (strict)"(error in=w711, "Value"=w671) -> (error out=w595:errorcluster)  [unwired: 1 in, 1 out]
    n210 = property on="Base A Level" class="Arr (strict)"(error in=w595, "Value"=w723) -> (error out=w594:errorcluster)  [unwired: 1 in, 1 out]
    n211 = disable-structure shown="Enabled" {
      disable-tunnel: w594 -> [w741 _]
      disable-tunnel: [w740 _] -> w645
      frame Disabled {
        n212 = property on="Base A Level" class="Arr (strict)"(error in=w741) -> (error out=w732:errorcluster, "Value"=w738:dbl[])  [unwired: 1 in, 1 out]
        n213 = property on="Base Color" class="Arr (strict)"(error in=w732) -> (error out=w731:errorcluster, "Value"=w739:u32[])  [unwired: 1 in, 1 out]
        n214 = property on="Level Composition" class="Arr (strict)"(error in=w731) -> (error out=w735:errorcluster, "Value"=w733:string[])  [unwired: 1 in, 1 out]
        n215 = property on="Base R Level" class="Arr (strict)"(error in=w735) -> (error out=w734:errorcluster, "Value"=w737:dbl[])  [unwired: 1 in, 1 out]
        n216 = CPU Information() -> (4:w736:i32)  [unwired: 3 out]
        n217 = for {
          workers-P: w736 -> [_]
          tunnel: w738 -> [w749] mode=indexing
          tunnel: w739 -> [w742] mode=indexing
          tunnel: [w746] -> w740
          tunnel: w737 -> [w748] mode=indexing
          tunnel: w734 -> [w745]
          tunnel: w733 -> [w743] mode=indexing
          i -> [w750]
          n218 = To Unsigned Long Integer(number=w750) -> (unsigned 32bit integer=w744:u32)
          n219 = disable-structure shown="無効" {
            disable-tunnel: w744 -> [w753 _]
            disable-tunnel: w743 -> [w752 _]
            disable-tunnel: w742 -> [w751 _]
            frame Disabled {
              n220 = property on="Time Graph Profile" class="XYGraph (strict)"("Active Plot"=w753, "Plot.Fill/Pt. Color"=w751, "Plot.Plot Name"=w752) -> ()  [unwired: 2 in, 2 out]
              n221 = property on="CP Graph Profile" class="XYGraph (strict)"("Active Plot"=w753, "Plot.Fill/Pt. Color"=w751, "Plot.Plot Name"=w752) -> ()  [unwired: 2 in, 2 out]
            }
            frame Enabled {
            }
          }
          n222 = property on="Data Histogram" class="XYGraph (strict)"(error in=w745, "Active Cursor"=w744, "Cursor.Cursor X"=w749, "Cursor.Cursor Color"=w742) -> (error out=w747:errorcluster)  [unwired: 1 in, 1 out]
          n223 = property on="Time Graph" class="XYGraph (strict)"(error in=w747, "Active Cursor"=w744, "Cursor.Cursor Y"=w748, "Cursor.Cursor Color"=w742) -> (error out=w746:errorcluster)  [unwired: 1 in, 1 out]
        }
      }
      frame Enabled {
      }
    }
    n224 = property on="BS Table Tag" class="Arr (strict)"(error in=w645) -> (error out=w644:errorcluster, "Value"=w692:string[])  [unwired: 1 in, 1 out]
    n225 = property on="BS Table" class="Tbl (strict)"(error in=w644) -> (error out=w643:errorcluster, "Value"=w693:string[][])  [unwired: 1 in, 1 out]
    n226 = call "Signal Table Anal.vi"("error in (no error)"=w643, "Signal Table"=w693, "Signal Tag"=w692) -> ("RR"=w689:i32[], "AR"=w691:i32[], "error out"=w642:errorcluster)  [unwired: 3 in, 3 out]
    n227 = property on="AR#" class="Arr (strict)"(error in=w642) -> (error out=w641:errorcluster, "Value"=w690:i32[])  [unwired: 1 in, 1 out]
    n228 = property on="RR#" class="Arr (strict)"(error in=w641) -> (error out=w640:errorcluster, "Value"=w688:i32[])  [unwired: 1 in, 1 out]
    n229 = Build Array (concatenate)(w689, w688) -> (w687:i32[])
    n230 = Build Array (concatenate)(w691, w690) -> (w587:i32[])
    n231 = Array Size(array=w587) -> (size(s)=w586:i32)
    n232 = property on="AR#" class="Arr (strict)"(error in=w640, "Value"=w587) -> (error out=w639:errorcluster)  [unwired: 1 in, 1 out]
    n233 = property on="RR#" class="Arr (strict)"(error in=w639, "Value"=w687) -> (error out=w588:errorcluster)  [unwired: 1 in, 1 out]
    n234 = property on="AR T#" class="DigNum (strict)"(error in=w588, "Value"=w586) -> (error out=w569:errorcluster)  [unwired: 1 in, 1 out]
    n235 = property on="Tag cluster_B" class="Clust (strict)"(error in=w569) -> (error out=w570:errorcluster, "Value"=w568:T7)  [unwired: 1 in, 1 out]
    n236 = property on="LCP Table" class="Tbl (strict)"(error in=w570) -> (error out=w622:errorcluster, "Value"=w695:string[][])  [unwired: 1 in, 1 out]
    n237 = property on="LSP Table" class="Tbl (strict)"(error in=w622) -> (error out=w621:errorcluster, "Value"=w694:string[][])  [unwired: 1 in, 1 out]
    n238 = property on="Level Composition" class="Arr (strict)"(error in=w621) -> (error out=w623:errorcluster, "Value"=w625:string[])  [unwired: 1 in, 1 out]
    n239 = property on="Cutted Sample Sequence" class="Str"(error in=w623) -> (error out=w565:errorcluster, "Value"=w624:string)  [unwired: 1 in, 1 out]
    n240 = property on="LAP Table" class="Tbl (strict)"(error in=w565) -> (error out=w564:errorcluster, "Value"=w566:string[][])  [unwired: 1 in, 1 out]
    n241 = call "LCP table array ans.vi"("LSP Table"=w694, "error in (no error)"=w564, "LAP Table"=w566, "LCP Table"=w695, "Tag cluster_B"=w568) -> ("error out"=w562:errorcluster, "LSPX_C2"=w626:T37, "LSPX_C1"=w619:T5, "LCPX_C1"=w620:T6, "LCPX_CZ"=w563:T1)  [unwired: 2 in]
    n242 = call "LC_Read_Number.vi"("Cutted Sample Sequence"=w624, "Level Composition"=w625, "LSPX_C2"=w626) -> ("Assigned#_CL"=w567:T4)  [unwired: 8 in]
    n243 = property on="LCPX_CZ" class="Clust (strict)"(error in=w562, "Value"=w563) -> (error out=w561:errorcluster)  [unwired: 1 in, 1 out]
    n244 = property on="LCPX_C1" class="Clust (strict)"(error in=w561, "Value"=w620) -> (error out=w618:errorcluster)  [unwired: 1 in, 1 out]
    n245 = property on="LSPX_C1" class="Clust (strict)"(error in=w618, "Value"=w619) -> (error out=w617:errorcluster)  [unwired: 1 in, 1 out]
    n246 = property on="Assigned#_CL" class="Clust (strict)"(error in=w617, "Value"=w567) -> (error out=w616:errorcluster)  [unwired: 1 in, 1 out]
    n247 = property on="Assigned#_CL" class="Clust (strict)"(error in=w616) -> (error out=w560:errorcluster, "Value"=w615:T4)  [unwired: 1 in, 1 out]
    n248 = property on="LCPX_CZ" class="Clust (strict)"(error in=w560) -> (error out=w558:errorcluster, "Value"=w559:T1)  [unwired: 1 in, 1 out]
    n249 = property on="LCPZ" class="Clust (strict)"(error in=w558) -> (error out=w557:errorcluster, "Value"=w556:T1)  [unwired: 1 in, 1 out]
    n250 = property on="LSP_C1" class="Clust (strict)"(error in=w557) -> (error out=w611:errorcluster, "Value"=w614:T9)  [unwired: 1 in, 1 out]
    n251 = property on="LSP_C2" class="Clust (strict)"(error in=w611) -> (error out=w610:errorcluster, "Value"=w612:T4)  [unwired: 1 in, 1 out]
    n252 = property on="LSPX_C1" class="Clust (strict)"(error in=w610) -> (error out=w609:errorcluster, "Value"=w613:T5)  [unwired: 1 in, 1 out]
    n253 = call "BSD Data accumlation.vi"("Assigned#_CL"=w615, "LSPX_C1"=w613, "LCPX_CZ"=w559, "error in (no error)"=w609, "LSP_C2 before"=w612, "LSP_C1 before"=w614, "LCPZ before"=w556) -> ("error out"=w555:errorcluster, "LSP_C2 after"=w585:T4, "LSP_C1 after"=w584:T9, "LCPZ after"=w553:T1)  [unwired: 1 in]
    n254 = Unbundle(w584) -> ("Seq SNo"=w583:i32[])  [unwired: 5 out]
    n255 = Array Size(array=w583) -> (size(s)=w582:i32)
    n256 = property on="LCPZ" class="Clust (strict)"(error in=w555, "Value"=w553) -> (error out=w554:errorcluster)  [unwired: 1 in, 1 out]
    n257 = property on="LSP_C1" class="Clust (strict)"(error in=w554, "Value"=w584) -> (error out=w589:errorcluster)  [unwired: 1 in, 1 out]
    n258 = property on="LSP_C2" class="Clust (strict)"(error in=w589, "Value"=w585) -> (error out=w581:errorcluster)  [unwired: 1 in, 1 out]
    n259 = property on="Long Signal#" class="DigNum (strict)"(error in=w581, "Value"=w582) -> (error out=w580:errorcluster)  [unwired: 1 in, 1 out]
    n260 = property on="GR data" class="Clust (strict)"(error in=w580) -> (error out=w716:errorcluster, "Value"=w722:T20)  [unwired: 1 in, 1 out]
    n261 = Unbundle(w722) -> ("Time Graph"=w721:cluster{"time":dbl[], "current":dbl[]}[], "CP Graph"=w720:cluster{i32[], dbl[]}[], "CP Graph Profile"=w719:cluster{i32[], dbl[]}[], "Time Graph Profile"=w718:cluster{"time":dbl[], dbl[]}[], "Plot Graph"=w717:dbl[][])  [unwired: 1 out]
    n262 = property on="Time Graph" class="XYGraph (strict)"(error in=w716, "Value"=w721) -> (error out=w715:errorcluster)  [unwired: 1 in, 1 out]
    n263 = property on="CP Graph" class="XYGraph (strict)"(error in=w715, "Value"=w720) -> (error out=w714:errorcluster)  [unwired: 1 in, 1 out]
    n264 = property on="CP Graph Profile" class="XYGraph (strict)"(error in=w714, "Value"=w719) -> (error out=w713:errorcluster)  [unwired: 1 in, 1 out]
    n265 = property on="Time Graph Profile" class="XYGraph (strict)"(error in=w713, "Value"=w718) -> (error out=w712:errorcluster)  [unwired: 1 in, 1 out]
    n266 = property on="Plot Graph" class="IntGraph (strict)"(error in=w712, "Value"=w717) -> (error out=w590:errorcluster)  [unwired: 1 in, 1 out]
    n267 = property on="AR T#" class="DigNum (strict)"(error in=w590) -> (error out=w632:errorcluster, "Value"=w638:i32)  [unwired: 1 in, 1 out]
    n268 = property on="Long Signal#" class="DigNum (strict)"(error in=w632) -> (error out=w631:errorcluster, "Value"=w636:i32)  [unwired: 1 in, 1 out]
    n269 = property on="AR BN#" class="Arr (strict)"(error in=w631) -> (error out=w630:errorcluster, "Value"=w637:i32[])  [unwired: 1 in, 1 out]
    n270 = property on="Right Read MIN" class="DigNum (strict)"(error in=w630) -> (error out=w629:errorcluster, "Value"=w635:i32)  [unwired: 1 in, 1 out]
    n271 = call "Signal Assembly Result Cluster.vi"("Right Read MIN"=w635, "AR BN#"=w637, "Long Signal#"=w636, "AR T#"=w638) -> ("RR MIN Over S#"=w633:i32, "Total assembly C"=w634:T24)  [unwired: 6 in]
    n272 = property on="Total assembly C" class="Clust (strict)"(error in=w629, "Value"=w634) -> (error out=w628:errorcluster)  [unwired: 1 in, 1 out]
    n273 = property on="RR MIN Over S#" class="DigNum (strict)"(error in=w628, "Value"=w633) -> (error out=w627:errorcluster)  [unwired: 1 in, 1 out]
    n274 = Get Date/Time In Seconds() -> (seconds since 1Jan1904=w703:timestamp)
    n275 = Format Date/Time String(time format string (%c)="%d:%H:%M:%S" ("時間形式文字列（%c）"), seconds (now)=w703) -> (date/time string=w700:string)  [unwired: 1 in]
    n276 = property on="after" class="Str"(error in=w627, "Value"=w700) -> (error out=w698:errorcluster)  [unwired: 1 in, 1 out]
    n277 = property on="before" class="Str"(error in=w698) -> (error out=w701:errorcluster, "Value"=w702:string)  [unwired: 1 in, 1 out]
    n278 = property on="after" class="Str"(error in=w701) -> (error out=w677:errorcluster, "Value"=w696:string)  [unwired: 1 in, 1 out]
    n279 = call "before and after.vi"("エラー入力"=w677, "after"=w696, "Before"=w702) -> ("エラー出力"=w697:errorcluster, "Anal Time"=w699:string)  [unwired: 7 in]
    n280 = property on="Anal Time" class="Str"(error in=w697, "Value"=w699) -> (error out=w597:errorcluster)  [unwired: 1 in, 1 out]
    n281 = property on="TDMS Tpath" class="Ref (strict)"(error in=w597) -> (error out=w575:errorcluster, "Value"=w678:refnum<k34>)  [unwired: 1 in, 1 out]
    n282 = property on="Table cluster_B" class="Clust (strict)"(error in=w575) -> (error out=w574:errorcluster, "Value"=w576:T3)  [unwired: 1 in, 1 out]
    n283 = property on="Tag cluster_B" class="Clust (strict)"(error in=w574) -> (error out=w596:errorcluster, "Value"=w552:T7)  [unwired: 1 in, 1 out]
    n284 = call "BNAL TDMS save table_MS.vi"("error in"=w596, "Tag cluster_B"=w552, "Table cluster_B"=w576, "TDMSファイル入力"=w678) -> ("error out"=w680:errorcluster, "A TDMSファイル出力"=w679:refnum<k34>)  [unwired: 6 in]
    n285 = property on="TDMS Tpath" class="Ref (strict)"(error in=w680, "Value"=w679) -> (error out=w646:errorcluster)  [unwired: 1 in, 1 out]
  }
  n286 = property on="AR T#" class="DigNum (strict)"("Value"=0 ("AR T#")) -> ()  [unwired: 2 in, 2 out]
  n287 = property on="LCPX_CZ" class="Clust (strict)"("Value"=w95) -> ()  [unwired: 2 in, 2 out]
  n288 = property on="LCPZ" class="Clust (strict)"("Value"=w95) -> ()  [unwired: 2 in, 2 out]
  n289 = property on="Cutted Sample Sequence" class="Str"(error in=w106) -> (error out=w136:errorcluster, "Value"=w130:string)  [unwired: 1 in, 1 out]
  n290 = property on="Right Read MIN" class="DigNum (strict)"(error in=w136) -> (error out=w144:errorcluster, "Value"=w131:i32)  [unwired: 1 in, 1 out]
  n291 = property on="LSP_C1" class="Clust (strict)"(error in=w144) -> (error out=w148:errorcluster, "Value"=w132:T9)  [unwired: 1 in, 1 out]
  n292 = Unbundle(w132) -> ("5’→3'"=w143:bool[], "Seq SNo"=w133:i32[], "Seq ENo"=w134:i32[], "Mx Right No"=w135:i32[])  [unwired: 2 out]
  n293 = call "BNAL assembly.vi"("Right Read MIN"=w131, "Mx Right No"=w135, "Seq ENo"=w134, "Seq SNo"=w133, "Cutted Sample Sequence"=w130) -> ("Long Signal#"=w145:i32, "Long Assembly"=w147:bool[][])  [unwired: 5 in]
  n294 = property on="Long Assembly" class="Arr (strict)"(error in=w148, "Value"=w147) -> (error out=w149:errorcluster)  [unwired: 1 in, 1 out]
  n295 = Array Size(array=w143) -> (size(s)=w137:i32)
  n296 = property on="Long Signal#" class="DigNum (strict)"(error in=w149, "Value"=w145) -> (error out=w156:errorcluster)  [unwired: 1 in, 1 out]
  n297 = for {
    N: w137 -> [_]
    tunnel: w143 -> [w758] mode=indexing
    shift-right: [w754] -> w138
    shift-left: 0 -> [w755]
    n298 = Equal?(x=w758, y=TRUE) -> (x = y?=w756:bool)
    n299 = case shown="False" w756 {
      tunnel: w755 -> [w759 w761]
      tunnel: [w759 w760] -> w754
      frame False {
      }
      frame True {
        n300 = Increment(x=w761) -> (x+1=w760:i32)
      }
    }
  }
  n301 = property on="Long Assembly" class="Arr (strict)"(error in=w156) -> (error out=w150:errorcluster, "Value"=w146:bool[][])  [unwired: 1 in, 1 out]
  n302 = call "Signal Count Assembly.vi"("Long Assembly"=w146) -> ("S#"=w128:i32, "RR#"=w127:i32, "Covered?"=w142:bool, "Total BC"=w126:bool[], "coverage [%]"=w140:dbl, "Total Base CP"=w141:i32)  [unwired: 5 in]
  n303 = Divide(x=w138, y=w137) -> (x/y=w139:dbl)
  n304 = property on="Total Base CP" class="DigNum (strict)"(error in=w150, "Value"=w141) -> (error out=w151:errorcluster)  [unwired: 1 in, 1 out]
  n305 = property on="Total BC" class="Arr (strict)"(error in=w151, "Value"=w126) -> (error out=w152:errorcluster)  [unwired: 1 in, 1 out]
  n306 = property on="Covered?" class="Bool (strict)"(error in=w152, "Value"=w142) -> (error out=w153:errorcluster)  [unwired: 1 in, 1 out]
  n307 = property on="RR#" class="DigNum (strict)"(error in=w153, "Value"=w127) -> (error out=w129:errorcluster)  [unwired: 1 in, 1 out]
  n308 = property on="S#" class="DigNum (strict)"(error in=w129, "Value"=w128) -> (error out=w154:errorcluster)  [unwired: 1 in, 1 out]
  n309 = property on="coverage [%]" class="DigNum (strict)"(error in=w154, "Value"=w140) -> (error out=w155:errorcluster)  [unwired: 1 in, 1 out]
  n310 = property on="5’→3'" class="DigNum (strict)"(error in=w155, "Value"=w139) -> (error out=w124:errorcluster)  [unwired: 1 in, 1 out]
  n311 = property on="noise MAX" class="DigNum (strict)"(error in=w124) -> (error out=w161:errorcluster, "Value"=w171:i32)  [unwired: 1 in, 1 out]
  n312 = property on="AR#" class="Arr (strict)"(error in=w161) -> (error out=w160:errorcluster, "Value"=w181:i32[])  [unwired: 1 in, 1 out]
  n313 = property on="RR#" class="Arr (strict)"(error in=w160) -> (error out=w180:errorcluster, "Value"=w182:i32[])  [unwired: 1 in, 1 out]
  n314 = call "RR Read number including repeat.vi"("noise MAX"=w171, "RR Read No"=w182) -> ("RR %"=w166:dbl[], "RR N#"=w165:i32[], "最大値"=w170:i32, "Av n#"=w172:dbl, "Av RR n#bp"=w189:i32)  [unwired: 2 in, 3 out]
  n315 = call "Read number total including repeat.vi"("noise MAX"=w171, "Read No"=w181) -> ("AR %"=w168:dbl[], "AR N#"=w167:i32[], "AR T#"=w192:i32, "Av n#"=w173:dbl, "AR BN#"=w193:i32[], "Av n#bp"=w185:i32)  [unwired: 1 in, 3 out]
  n316 = property on="BR time [s]" class="DigNum (strict)"(error in=w180) -> (error out=w177:errorcluster, "Value"=w175:dbl)  [unwired: 1 in, 1 out]
  n317 = Divide(x=w185, y=w175) -> (x/y=w174:dbl)
  n318 = Divide(x=w189, y=w175) -> (x/y=w176:dbl)
  n319 = Bundle("AR N#"=w167, "AR %"=w168) -> (w163:cluster{"AR N#":i32[], "AR %":dbl[]})  [unwired: 1 in]
  n320 = Bundle("RR N#"=w165, "RR %"=w166) -> (w164:cluster{"RR N#":i32[], "RR %":dbl[]})  [unwired: 1 in]
  n321 = Multiply(x=w174, y=w162) -> (x*y=w184:dbl)
  n322 = Multiply(x=w176, y=w162) -> (x*y=w183:dbl)
  n323 = Build Array(w164, w163) -> (w169:cluster{"AR N#":i32[], "AR %":dbl[]}[])
  n324 = property on="Signal# Histogram" class="XYGraph (strict)"(error in=w177, "Value"=w169) -> (error out=w178:errorcluster)  [unwired: 1 in, 1 out]
  n325 = property on="Av R_Read N" class="DigNum (strict)"(error in=w178, "Value"=w173) -> (error out=w179:errorcluster)  [unwired: 1 in, 1 out]
  n326 = property on="Av N_Read N" class="DigNum (strict)"(error in=w179, "Value"=w172) -> (error out=w186:errorcluster)  [unwired: 1 in, 1 out]
  n327 = property on="Av n#bp" class="DigNum (strict)"(error in=w186, "Value"=w185) -> (error out=w187:errorcluster)  [unwired: 1 in, 1 out]
  n328 = property on="Av n# kbp/day" class="DigNum (strict)"(error in=w187, "Value"=w184) -> (error out=w188:errorcluster)  [unwired: 1 in, 1 out]
  n329 = property on="Av RRn# kbp/day" class="DigNum (strict)"(error in=w188, "Value"=w183) -> (error out=w190:errorcluster)  [unwired: 1 in, 1 out]
  n330 = property on="Av RR n#bp" class="DigNum (strict)"(error in=w190, "Value"=w189) -> (error out=w191:errorcluster)  [unwired: 1 in, 1 out]
  n331 = property on="MAX RR#" class="DigNum (strict)"(error in=w191, "Value"=w170) -> (error out=w159:errorcluster)  [unwired: 1 in, 1 out]
  n332 = property on="AR T#" class="DigNum (strict)"(error in=w159, "Value"=w192) -> (error out=w158:errorcluster)  [unwired: 1 in, 1 out]
  n333 = property on="AR BN#" class="Arr (strict)"(error in=w158, "Value"=w193) -> (error out=w157:errorcluster)  [unwired: 1 in, 1 out]
  n334 = property on="LSP_C1" class="Clust (strict)"(error in=w157) -> (error out=w198:errorcluster, "Value"=w201:T9)  [unwired: 1 in, 1 out]
  n335 = Unbundle(w201) -> ("Q value [x]"=w200:dbl[], "Signal Length [ms]"=w199:dbl[])  [unwired: 4 out]
  n336 = property on="MS_Total Con and T" class="Clust (strict)"("Value"=cluster{dbl[], dbl[], dbl[], dbl[], i32[]} {[], [], [], [], []} ("MS_Total Con and T")) -> ()  [unwired: 2 in, 2 out]
  n337 = call <vilib>:"Histogram.vi"("intervals"=50, "X"=w200) -> ("Histogram Graph"=w204:T26)  [unwired: 6 in, 3 out]
  n338 = call <vilib>:"Histogram.vi"("intervals"=50, "X"=w199) -> ("Histogram Graph"=w205:T26)  [unwired: 6 in, 3 out]
  n339 = property on="Q_Histogram" class="XYGraph (strict)"(error in=w198, "Value"=w204) -> (error out=w206:errorcluster)  [unwired: 1 in, 1 out]
  n340 = property on="Time Histogram" class="XYGraph (strict)"(error in=w206, "Value"=w205) -> (error out=w105:errorcluster)  [unwired: 1 in, 1 out]
  n341 = property on="LCPZ" class="Clust (strict)"(error in=w105) -> (error out=w104:errorcluster, "Value"=w103:T1)  [unwired: 1 in, 1 out]
  n342 = Unbundle(w103) -> ("Relative Averaged Data"=w115:dbl[], "Time"=w114:dbl[], "AS IDX"=w116:i32[], "Signal Intensity [pA]"=w110:dbl[], "LA_Relative Averaged Data"=w102:dbl[], "LA_Time"=w101:dbl[], "MS_IDX"=w100:i32[], "LA_Signal Intensity [pA]"=w99:dbl[])
  n343 = call "bnal PLOT_MS.vi"("AS IDX"=w116, "error in"=w104, "Signal Intensity [pA]"=w110, "Time"=w114, "Relative Averaged Data"=w115) -> ("error out"=w98:errorcluster, "R Con H"=w111:dbl[][], "Plot_C"=w112:T38, "Plot Graph"=w113:T39)  [unwired: 3 in]
  n344 = call "bnal PLOT_NS.vi"("AS IDX"=w100, "error in"=w98, "Signal Intensity [pA]"=w99, "Time"=w101, "Relative Averaged Data"=w102) -> ("error out"=w97:errorcluster, "R Con H"=w94:dbl[][], "Plot_C"=w64:T38, "Plot Graph"=w96:T39)  [unwired: 3 in]
  n345 = Unbundle(w112) -> ("Count Graph"=w245:cluster{i32[], i32[]}, "Total Con and T"=w246:cluster{dbl[], dbl[], dbl[], dbl[], i32[]}, "GAT"=w247:T40)
  n346 = Unbundle(w247) -> ("Value"=w234:T14)  [unwired: 2 out]
  "GAF" <- w234
  n347 = Unbundle(w96) -> ("Plot Graph"=w92:dbl[][], "N_Grpah"=w93:dbl[][])  [unwired: 1 out]
  n348 = Unbundle(w113) -> ("Plot Graph"=w248:dbl[][], "N_Grpah"=w244:dbl[][], "Abs_Graph"=w243:dbl[][])
  n349 = Unbundle(w234) -> ("Abs MIN"=w236:dbl, "Abs Multiplier"=w250:dbl, "Abs MAX"=w237:dbl, "P MIN"=w239:dbl, "P Multiplier"=w238:dbl, "P MAX"=w240:dbl, "X MAX"=w241:dbl)
  n350 = Unbundle(w64) -> ("Count Graph"=w62:cluster{i32[], i32[]}, "Total Con and T"=w61:cluster{dbl[], dbl[], dbl[], dbl[], i32[]})  [unwired: 1 out]
  n351 = call <vilib>:"Histogram.vi"("intervals"=50, "X"=w110) -> ("Histogram Graph"=→"I Histogram":T26)  [unwired: 6 in, 3 out]
  n352 = Multiply(x=w250, y=w237) -> (x*y=w249:dbl)
  n353 = property on="Total C Plot" class="IntGraph (strict)"(error in=w97, "Value"=w248) -> (error out=w251:errorcluster)  [unwired: 1 in, 1 out]
  n354 = property on="Total NGraph" class="IntGraph (strict)"(error in=w251, "Value"=w244) -> (error out=w230:errorcluster)  [unwired: 1 in, 1 out]
  n355 = property on="Count Graph" class="XYGraph (strict)"(error in=w230, "Value"=w245) -> (error out=w231:errorcluster)  [unwired: 1 in, 1 out]
  n356 = property on="Total Con and T" class="Clust (strict)"(error in=w231, "Value"=w246) -> (error out=w232:errorcluster)  [unwired: 1 in, 1 out]
  n357 = property on="R Con H" class="Arr (strict)"(error in=w232, "Value"=w111) -> (error out=w233:errorcluster)  [unwired: 1 in, 1 out]
  n358 = property on="Total AGraph" class="IntGraph (strict)"(error in=w233, "Value"=w243) -> (error out=w235:errorcluster)  [unwired: 1 in, 1 out]
  n359 = property on="Total AGraph" class="IntGraph (strict)"(error in=w235, "YScale.Offset"=w236, "YScale.Multiplier"=w250, "YScale.Minimum"=w236, "YScale.Maximum"=w249, "XScale.Maximum"=w241) -> (error out=w242:errorcluster)  [unwired: 1 in, 1 out]
  n360 = property on="Total NGraph" class="IntGraph (strict)"(error in=w242, "YScale.Offset"=w239, "YScale.Multiplier"=w238, "YScale.Minimum"=w239, "YScale.Maximum"=w240, "XScale.Maximum"=w241) -> (error out=w91:errorcluster)  [unwired: 1 in, 1 out]
  n361 = property on="R Con H_MS" class="Arr (strict)"(error in=w91, "Value"=w94) -> (error out=w90:errorcluster)  [unwired: 1 in, 1 out]
  n362 = property on="Total C Plot_MS" class="Arr (strict)"(error in=w90, "Value"=w92) -> (error out=w89:errorcluster)  [unwired: 1 in, 1 out]
  n363 = property on="Total NGraph_MS" class="IntGraph (strict)"(error in=w89, "Value"=w93) -> (error out=w60:errorcluster)  [unwired: 1 in, 1 out]
  n364 = property on="MS_Count Graph" class="XYGraph (strict)"(error in=w60, "Value"=w62) -> (error out=w59:errorcluster)  [unwired: 1 in, 1 out]
  n365 = property on="MS_Total Con and T" class="Clust (strict)"(error in=w59, "Value"=w61) -> (error out=w58:errorcluster)  [unwired: 1 in, 1 out]
  n366 = call <vilib>:"Clear Errors.vi"("error in (no error)"=w58, "specific error code to clear (0: all)"=-2501) -> ("error out"=w226:errorcluster)  [unwired: 4 in, 1 out]
  n367 = property on="LSP_C2" class="Clust (strict)"(error in=w226) -> (error out=w225:errorcluster, "Value"=w218:T4)  [unwired: 1 in, 1 out]
  n368 = property on="Level Composition" class="Arr (strict)"(error in=w225) -> (error out=w252:errorcluster, "Value"=w224:string[])  [unwired: 1 in, 1 out]
  n369 = property on="Cutted Sample Sequence" class="Str"(error in=w252) -> (error out=w216:errorcluster, "Value"=w223:string)  [unwired: 1 in, 1 out]
  n370 = call "BNAL RADAR graph Formation.vi"("Cutted Sample Sequence"=w223, "Level Composition"=w224, "Assigned#_CL"=w218) -> ("Base_Tag_Array"=w75:string[], "Base_Com_Array"=w76:i32[], "Table Cluster"=w219:T41, "Radar graph cluster"=w222:T42)  [unwired: 5 in]
  n371 = Unbundle(w222) -> ("Radar Plot"=w221:picture, "Radar Plot"=w220:picture)  [unwired: 1 out]
  n372 = Unbundle(w219) -> ("Mono Table"=w215:string[][], "Mono Table"=w214:string[][], "Mono Table"=w213:string[][])
  n373 = property on="All Radar_X" class="Pict"(error in=w216, "Value"=w221) -> (error out=w255:errorcluster)  [unwired: 1 in, 1 out]
  n374 = property on="All Radar Plot_XX" class="Pict"(error in=w255, "Value"=w220) -> (error out=w217:errorcluster)  [unwired: 1 in, 1 out]
  n375 = property on="Mono Table" class="Tbl (strict)"(error in=w217, "Value"=w215) -> (error out=w253:errorcluster)  [unwired: 1 in, 1 out]
  n376 = property on="Di Table" class="Tbl (strict)"(error in=w253, "Value"=w214) -> (error out=w254:errorcluster)  [unwired: 1 in, 1 out]
  n377 = property on="Tri Table" class="Tbl (strict)"(error in=w254, "Value"=w213) -> (error out=w69:errorcluster)  [unwired: 1 in, 1 out]
  n378 = property on="Base_Com_Array" class="Arr (strict)"(error in=w69, "Value"=w76) -> (error out=w68:errorcluster)  [unwired: 1 in, 1 out]
  n379 = property on="Base_Tag_Array" class="Arr (strict)"(error in=w68, "Value"=w75) -> (error out=w22:errorcluster)  [unwired: 1 in, 1 out]
  "error out 2" <- w22
  n380 = for {
    N: 5 -> [_]
    shift-right: [w776] -> w467
    shift-left: w22 -> [w780]
    tunnel: [w762] -> w23 mode=indexing
    i -> [w779]
    n381 = case shown="4" w779 {
      tunnel: [T22."Plot" ("Control_2") T22."Assembly" ("Control_2") T22."Model" ("Control_2") T22."Radar" ("Control_2") T22."Plot_MS" ("Control_2")] -> w763
      tunnel: w780 -> [w786 w790 w792 w796 w800]
      tunnel: [w786 w790 w792 w796 w800] -> w778
      tunnel: [w784 w789 w793 w797 w799] -> w770
      tunnel: w779 -> [w785 w788 w794 w798 w802]
      frame 0, Default {
        n382 = Number To Decimal String(number=w785) -> (decimal integer string=w784:string)  [unwired: 1 in]
      }
      frame 1 {
        n383 = Number To Decimal String(number=w788) -> (decimal integer string=w789:string)  [unwired: 1 in]
      }
      frame 2 {
        n384 = Number To Decimal String(number=w794) -> (decimal integer string=w793:string)  [unwired: 1 in]
      }
      frame 3 {
        n385 = Number To Decimal String(number=w798) -> (decimal integer string=w797:string)  [unwired: 1 in]
      }
      frame 4 {
        n386 = Number To Decimal String(number=w802) -> (decimal integer string=w799:string)  [unwired: 1 in]
      }
    }
    n387 = Concatenate Strings("Long" ("LG name"), w770) -> (w765:string)
    n388 = property on="Folder Path" class="Str"(error in=w778) -> (error out=w777:errorcluster, "Value"=w772:string)  [unwired: 1 in, 1 out]
    n389 = property on="Date" class="Str"(error in=w777) -> (error out=w767:errorcluster, "Value"=w771:string)  [unwired: 1 in, 1 out]
    n390 = property on="Right Read MIN" class="DigNum (strict)"(error in=w767) -> (error out=w766:errorcluster, "Value"=w768:i32)  [unwired: 1 in, 1 out]
    n391 = property on="FN#" class="Str" props=["Value"]() -> ()  [unwired: 2 in, 3 out]
    n392 = local write "Control_2"(w763) -> ()
    n393 = Number To Decimal String(number=w768) -> (decimal integer string=w774:string)  [unwired: 1 in]
    n394 = Concatenate Strings(w772, "\\" ("文字列"), w765, "_" ("文字列"), w774, w771, ".jpg" ("文字列")) -> (w762:string)
    n395 = Current VI's Path() -> (path=w781:path)
    n396 = String To Path(string=w762) -> (path=w782:path)
    n397 = call "Front Panel JPEG file converter.vi"("error in"=w766, "JPEG file name"=w782, "VI Path"=w781) -> ("error out"=w776:errorcluster)  [unwired: 8 in]
  }
  "Array" <- w23
  n398 = property on="Total C Plot" class="IntGraph (strict)"(error in=w467) -> (error out=w470:errorcluster, "Value"=w431:dbl[][])  [unwired: 1 in, 1 out]
  n399 = property on="Total NGraph" class="IntGraph (strict)"(error in=w470) -> (error out=w469:errorcluster, "Value"=w430:dbl[][])  [unwired: 1 in, 1 out]
  n400 = property on="Folder Path" class="Str"(error in=w469) -> (error out=w468:errorcluster, "Value"=w88:string)  [unwired: 1 in, 1 out]
  n401 = property on="Date" class="Str"(error in=w468) -> (error out=w427:errorcluster, "Value"=w87:string)  [unwired: 1 in, 1 out]
  n402 = property on="R Con H" class="Arr (strict)"(error in=w427) -> (error out=w426:errorcluster, "Value"=w428:dbl[][])  [unwired: 1 in, 1 out]
  n403 = call "Histogram Plot save.vi"("R Con H"=w428, "Date"=w87, "error in"=w426, "Normalized Plot Graph"=w430, "Plot Graph"=w431, "Folder Path"=w88) -> ("error out"=w84:errorcluster)  [unwired: 5 in]
  n404 = property on="Total C Plot_MS" class="Arr (strict)"(error in=w84) -> (error out=w83:errorcluster, "Value"=w86:dbl[][])  [unwired: 1 in, 1 out]
  n405 = property on="Total NGraph_MS" class="IntGraph (strict)"(error in=w83) -> (error out=w82:errorcluster, "Value"=w85:dbl[][])  [unwired: 1 in, 1 out]
  n406 = property on="R Con H_MS" class="Arr (strict)"(error in=w82) -> (error out=w81:errorcluster, "Value"=w80:dbl[][])  [unwired: 1 in, 1 out]
  n407 = call "Histogram Plot save_MS.vi"("R Con H"=w80, "Date"=w87, "error in"=w81, "Normalized Plot Graph"=w85, "Plot Graph"=w86, "Folder Path"=w88) -> ("error out"=w77:errorcluster)  [unwired: 5 in]
  n408 = property on="TDMS Tpath" class="Ref (strict)"(error in=w77) -> (error out=w74:errorcluster, "Value"=w79:refnum<k34>)  [unwired: 1 in, 1 out]
  n409 = property on="Base_Tag_Array" class="Arr (strict)"(error in=w74) -> (error out=w73:errorcluster, "Value"=w71:string[])  [unwired: 1 in, 1 out]
  n410 = property on="Base_Com_Array" class="Arr (strict)"(error in=w73) -> (error out=w72:errorcluster, "Value"=w70:i32[])  [unwired: 1 in, 1 out]
  n411 = call "LADAR value save VI.vi"("error in"=w72, "LL_Base_Com_Array"=w70, "LL_Base Tag_Array"=w71, "TDMSファイル入力"=w79) -> ("error out"=w24:errorcluster, "A TDMSファイル出力"=w78:refnum<k34>)  [unwired: 6 in]
  n412 = property on="TDMS Tpath" class="Ref (strict)"(error in=w24, "Value"=w78) -> (error out=w50:errorcluster)  [unwired: 1 in, 1 out]
  n413 = property on="Cutted Sample Sequence" class="Str"(error in=w50) -> (error out=w49:errorcluster, "Value"=w54:string)  [unwired: 1 in, 1 out]
  n414 = property on="Sample Sequence" class="Str"(error in=w49) -> (error out=w48:errorcluster, "Value"=w53:string)  [unwired: 1 in, 1 out]
  n415 = property on="Total Con and T" class="Clust (strict)"(error in=w48) -> (error out=w47:errorcluster, "Value"=w56:T19)  [unwired: 1 in, 1 out]
  n416 = property on="MS_Total Con and T" class="Clust (strict)"(error in=w47) -> (error out=w46:errorcluster, "Value"=w55:cluster{dbl[], dbl[], dbl[], dbl[], i32[]})  [unwired: 1 in, 1 out]
  n417 = property on="Date" class="Str"(error in=w46) -> (error out=w45:errorcluster, "Value"=w51:string)  [unwired: 1 in, 1 out]
  n418 = property on="Folder Path" class="Str"(error in=w45) -> (error out=w44:errorcluster, "Value"=w52:string)  [unwired: 1 in, 1 out]
  n419 = call "Depth count VI.vi"("MS_Total Con and T"=w55, "Date"=w51, "Total Con and T"=w56, "error in"=w44, "Folder Path"=w52, "Sample Sequence"=w53, "Cutted Sample Sequence"=w54) -> ("error out"=w57:errorcluster)  [unwired: 4 in]
  n420 = property on="S#" class="DigNum (strict)"(error in=w57) -> (error out=w358:errorcluster, "Value"=w376:i32)  [unwired: 1 in, 1 out]
  n421 = property on="MAX RR#" class="DigNum (strict)"(error in=w358) -> (error out=w357:errorcluster, "Value"=w375:i32)  [unwired: 1 in, 1 out]
  n422 = property on="RR#" class="DigNum (strict)"(error in=w357) -> (error out=w356:errorcluster, "Value"=w374:i32)  [unwired: 1 in, 1 out]
  n423 = property on="Av n#bp" class="DigNum (strict)"(error in=w356) -> (error out=w355:errorcluster, "Value"=w373:i32)  [unwired: 1 in, 1 out]
  n424 = property on="Av RRn# kbp/day" class="DigNum (strict)"(error in=w355) -> (error out=w354:errorcluster, "Value"=w372:dbl)  [unwired: 1 in, 1 out]
  n425 = property on="Av RR n#bp" class="DigNum (strict)"(error in=w354) -> (error out=w353:errorcluster, "Value"=w371:i32)  [unwired: 1 in, 1 out]
  n426 = property on="Av n# kbp/day" class="DigNum (strict)"(error in=w353) -> (error out=w352:errorcluster, "Value"=w370:dbl)  [unwired: 1 in, 1 out]
  n427 = property on="coverage [%]" class="DigNum (strict)"(error in=w352) -> (error out=w351:errorcluster, "Value"=w369:dbl)  [unwired: 1 in, 1 out]
  n428 = property on="5’→3'" class="DigNum (strict)"(error in=w351) -> (error out=w350:errorcluster, "Value"=w368:dbl)  [unwired: 1 in, 1 out]
  n429 = property on="Av N_Read N" class="DigNum (strict)"(error in=w350) -> (error out=w349:errorcluster, "Value"=w367:dbl)  [unwired: 1 in, 1 out]
  n430 = property on="Av R_Read N" class="DigNum (strict)"(error in=w349) -> (error out=w348:errorcluster, "Value"=w366:dbl)  [unwired: 1 in, 1 out]
  n431 = property on="RR MIN Over S#" class="DigNum (strict)"(error in=w348) -> (error out=w347:errorcluster, "Value"=w365:i32)  [unwired: 1 in, 1 out]
  n432 = property on="Total Base CP" class="DigNum (strict)"(error in=w347) -> (error out=w346:errorcluster, "Value"=w364:i32)  [unwired: 1 in, 1 out]
  n433 = property on="Covered?" class="Bool (strict)"(error in=w346) -> (error out=w345:errorcluster, "Value"=w363:bool)  [unwired: 1 in, 1 out]
  n434 = property on="Anal Time" class="Str"(error in=w345) -> (error out=w344:errorcluster, "Value"=w362:string)  [unwired: 1 in, 1 out]
  n435 = Current VI's Path() -> (path=w377:path)
  n436 = Strip Path(path=w377) -> (name=w378:string)  [unwired: 1 out]
  n437 = Bundle("Value"=w376, "Value"=w375, "Value"=w374, "Value"=w373, "Value"=w372, "Value"=w371, "Value"=w370, "Value"=w369, "Value"=w368, "Value"=w367, "Value"=w366, "Value"=w365, "Value"=w364, "Value"=w363, "Value"=w362) -> (w342:T43)  [unwired: 1 in]
  "B prep" <- w342
  n438 = call "GetFileCreationDate.vi"("File Path"=w377) -> ("File Created Date (UTC)"=w361:timestamp)  [unwired: 7 in, 1 out]
  n439 = Match Pattern(string=w378, regular expression=".vi" ("正規表現")) -> (before substring=w360:string)  [unwired: 1 in, 3 out]
  "BNAL Program" <- w360
  n440 = property on="SB_ANA" class="Clust (strict)"(error in=w344) -> (error out=w343:errorcluster, "Value"=w340:T25)  [unwired: 1 in, 1 out]
  n441 = property on="Total assembly C" class="Clust (strict)"(error in=w343) -> (error out=w338:errorcluster, "Value"=w341:T24)  [unwired: 1 in, 1 out]
  n442 = property on="TDMS Tpath" class="Ref (strict)"(error in=w338) -> (error out=w337:errorcluster, "Value"=w30:refnum<k34>)  [unwired: 1 in, 1 out]
  n443 = Format Date/Time String(time format string (%c)="%Y_%m%d_%H:%M:%S" ("時間形式文字列（%c）"), seconds (now)=w361) -> (date/time string=w359:string)  [unwired: 1 in]
  "BNAL Program Date" <- w359
  n444 = Bundle("name"=w360, "date/time string"=w359) -> (w339:T11)  [unwired: 1 in]
  "BNAL TD" <- w339
  n445 = call "BNAL Csave Preaparation VI.vi"("BNAL TD"=w339, "SB_ANA"=w340, "error in"=w337, "Total assembly C"=w341, "B prep"=w342, "TDMSファイル in"=w30) -> ("error out"=w37:errorcluster)  [unwired: 4 in, 1 out]
  n446 = property on="B_TDMS_Path" class="Path"(error in=w37) -> (error out=w36:errorcluster, "Value"=w31:path)  [unwired: 1 in, 1 out]
  n447 = property on="B_TDMS_Path_Temp" class="Path"(error in=w36) -> (error out=w35:errorcluster, "Value"=w27:path)  [unwired: 1 in, 1 out]
  n448 = Copy(8:w35, 10:w31, 11:w27) -> (0:w29:errorcluster)  [unwired: 2 in, 2 out]
  n449 = call "tdms_index_trans.vi"("B_TDMS_Path_Temp"=w27) -> ("path"=w26:path)  [unwired: 10 in]
  n450 = Delete(path (use dialog)=w27, entire hierarchy (F)=w25, error in=w29) -> (error out=w28:errorcluster)  [unwired: 2 in, 2 out]
  n451 = Delete(path (use dialog)=w26, entire hierarchy (F)=w25, error in=w28) -> (error out=w10:errorcluster)  [unwired: 2 in, 2 out]
  n452 = Unbundle(w10) -> ("status"=w11:bool)  [unwired: 2 out]
  n453 = property on="Locked" class="Bool (strict)"(error in=w10, "Value"=TRUE ("Locked")) -> (error out=→"error out":errorcluster)  [unwired: 1 in, 1 out]
  n454 = Request Deallocation(w11) -> ()
  "LSP_C2" <- w212
  "LCPX_C1" <- T30 {"Relative Averaged Data"=[], "Time"=[], "AS IDX"=[], "Abs Average"=[]} ("LCPX_C1")
  "LSPX_C1" <- T5 {"Q value [x]"=[], "Signal Length [ms]"=[], "5’→3'"=[], "Seq SNo"=[], "Seq ENo"=[], "Mx Right No"=[], "Signal Start [s]"=[], "S IDX"=[], "Signal End [s]"=[]} ("LSPX_C1")
  "Assigned#_CL" <- w212
